vi "Host_spb.vi"   [LabVIEW 2018]
uses:
  <vilib>/userdefined/High Color/nirio_resource_hc.ctl
  <instrlib>/niDMM/nidmm.llb/niDMM Function.ctl
  <instrlib>/niDMM/nidmm.llb/niDMM Resolution in Digits.ctl
  <instrlib>/niDCPower/nidcpower.llb/niDCPower Measurement Type.ctl
  <instrlib>/niDMM/nidmm.llb/niDMM Configure Measurement Digits.vi
  <vilib>/FPGAPlugInAG/PXI-7953R/niLvFpga_Open_PXI-7953R.vi
  <vilib>/rvi/interface/common/dynamic/niFpgaDynamicAddResources.vi
  <vilib>/FPGAPlugInAG/Dynamic/niLvFpga_Reset_Dynamic.vi
  <vilib>/FPGAPlugInAG/Dynamic/niLvFpga_Run_Dynamic.vi
  <vilib>/Utility/error.llb/Error Cluster From Error Code.vi
  <vilib>/rvi/errors/niLvFpgaAdjustHostInterfaceError.vi
  <vilib>/FPGAPlugInAG/Dynamic/niLvFpga_Abort_Dynamic.vi
  <vilib>/rvi/interface/nirviOpenFPGA/nirviOpenFPGA.xnode
  <vilib>/rvi/interface/nirviMethod/nirviMethod.xnode
  <vilib>/rvi/interface/nirviReadWriteControl/nirviReadWriteControl.xnode
  NiFpgaLv.dll
  <vilib>/rvi/interface/Simulation/niFpgaSimulationCallBeginRW.vi
  <vilib>/FPGAPlugInAG/Dynamic/niLvFpga_ReadFifo_Dynamic.vi
  <vilib>/rvi/errors/niLvFpgaMergeErrorWithErrorCode.vi
types:
  T1 = enum16{"open", "replace", "create", "open or create", "replace or create", "replace or create with confirmation"}
  T2 = typedef "niDMM Function.ctl" = enum16{"DC Volts", "AC Volts", "DC Current", "AC Current", "2-wire Resistance", "4-wire Resistance", "Diode", "Frequency", "Period", "AC Volts DC Coupled", "Capacitance", "Inductance", "Temperature"}
  T3 = typedef "niDMM Resolution in Digits.ctl" = dbl
  T4 = cluster{"Global Rectangle":i32[], "Contours":cluster{"Contour Type":u32, "ROI Type":u32, "Points":i32[]}[]}
  T5 = cluster{"Contour Type":u32, "ROI Type":u32, "Points":i32[]}[]
  T6 = cluster{"Contour Type":u32, "ROI Type":u32, "Points":i32[]}
  T7 = typedef "IMAQ Image.ctl" = refnum<image>
  T8 = enum16{"Configuration", "MUX", "RED PGA", "GREEN PGA", "BLUE PGA", "RED OFF", "GREEN OFF", "BLUE OFF"}
  T9 = typedef "Image Type" = u32
  T10 = typedef "niDCPower Measurement Type.ctl" = i32
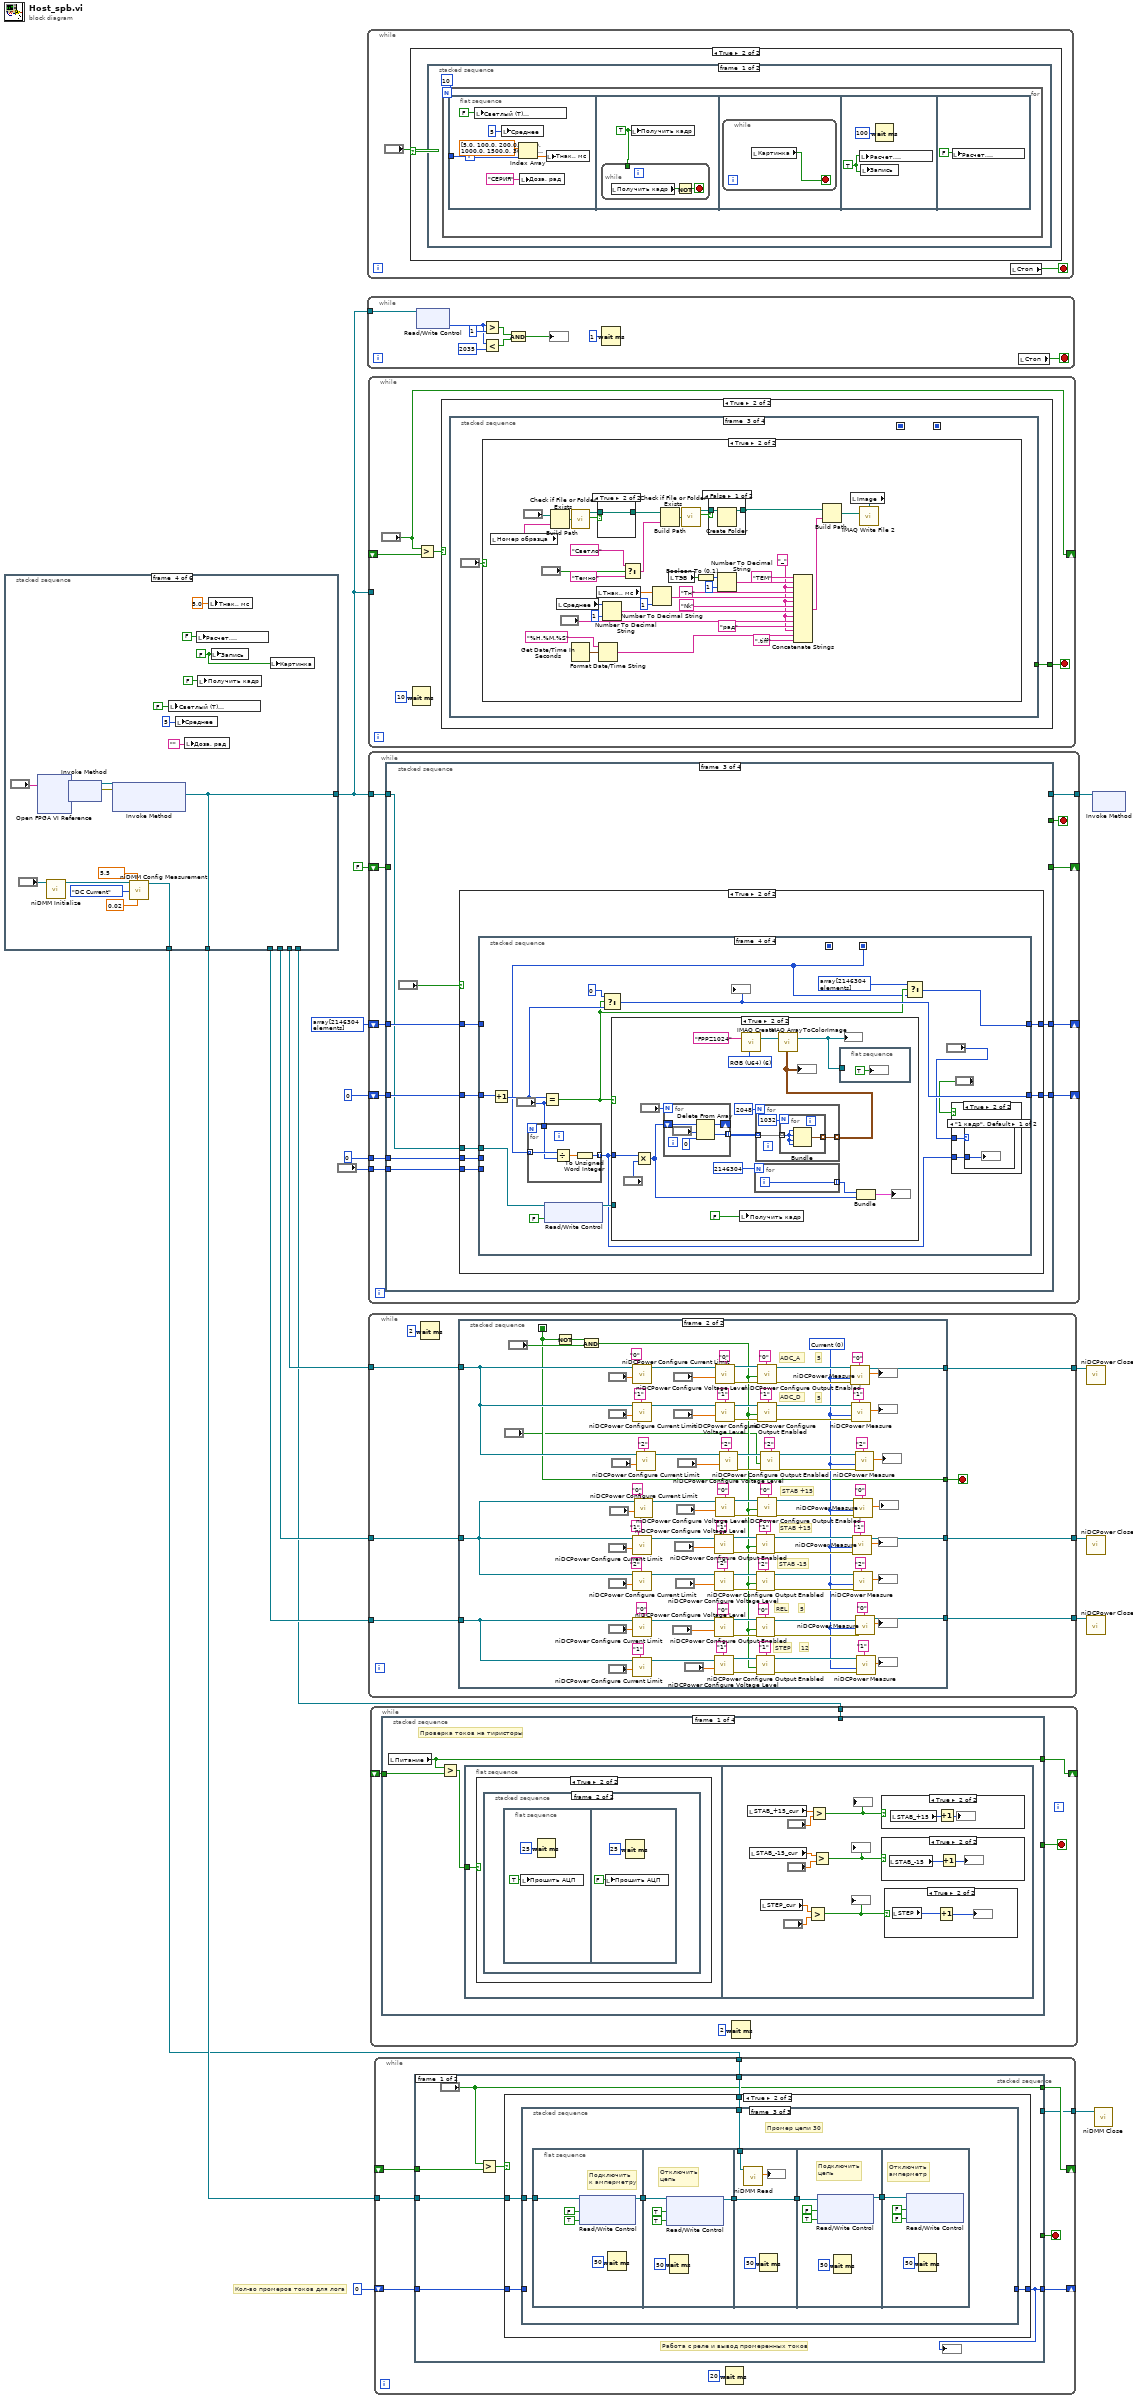
[diagram p0: block diagram]
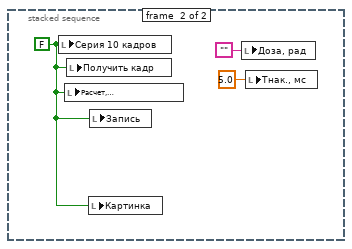
[diagram p3: hidden frame]
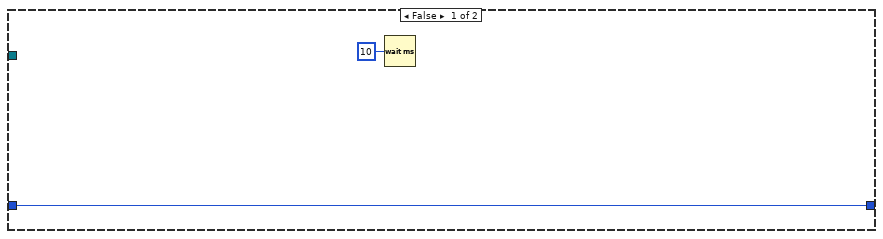
[diagram p4: hidden frame]
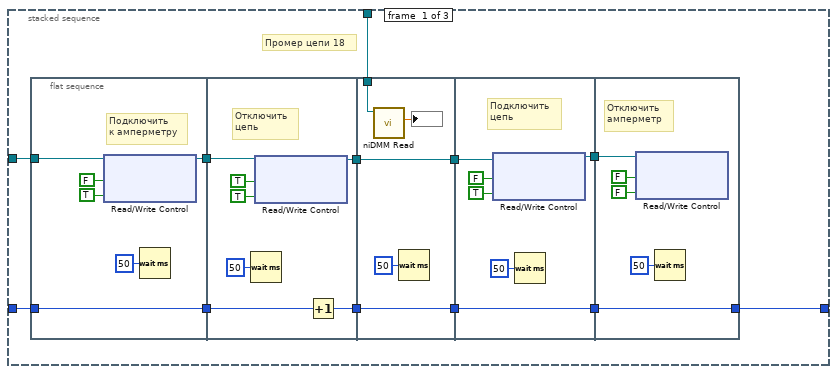
[diagram p5: hidden frame]
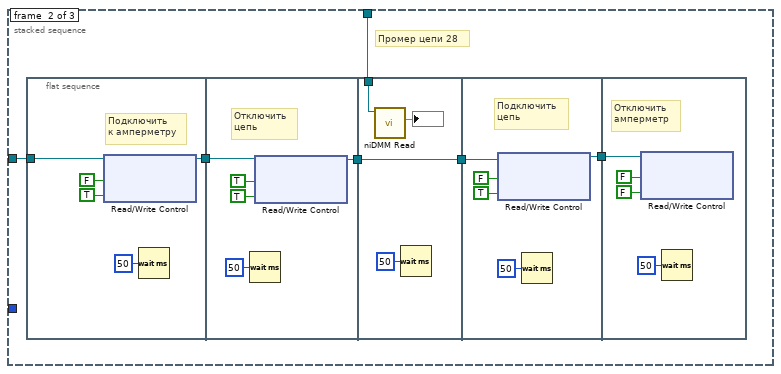
[diagram p6: hidden frame]
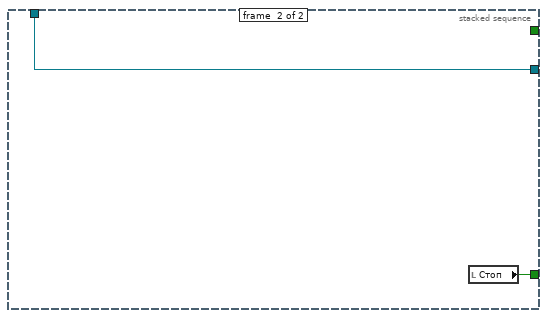
[diagram p7: hidden frame]
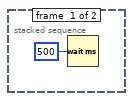
[diagram p9: hidden frame]
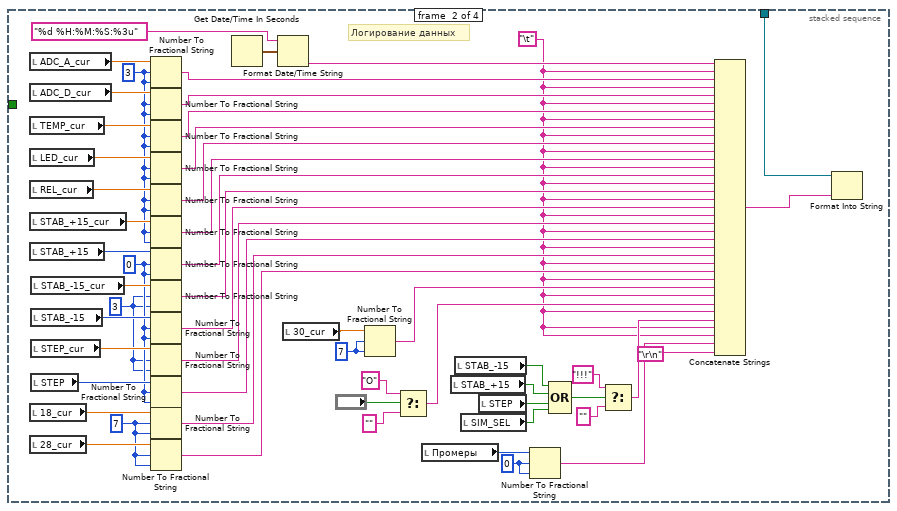
[diagram p13: hidden frame]
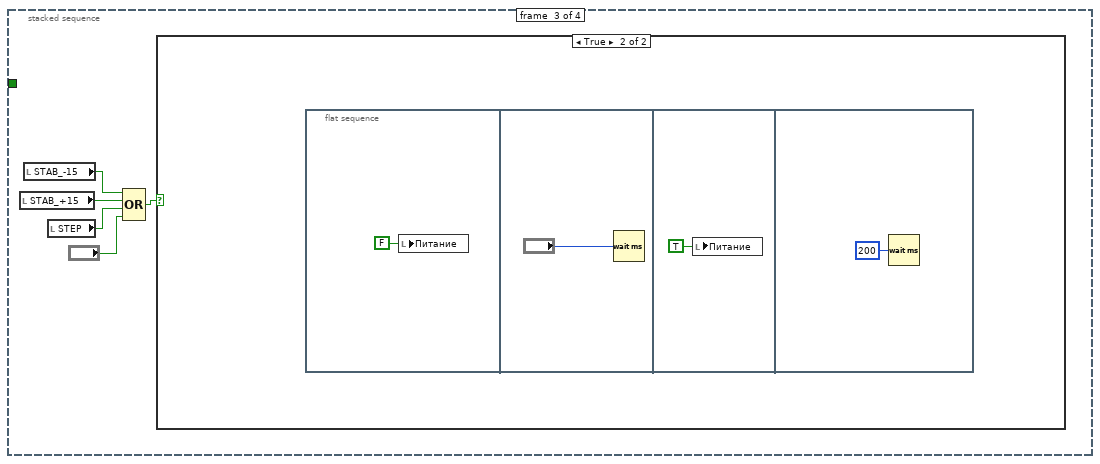
[diagram p14: hidden frame]
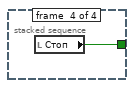
[diagram p16: hidden frame]
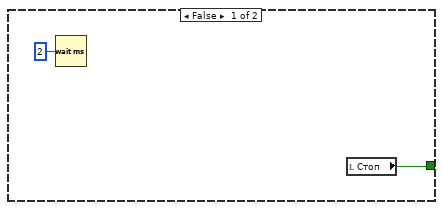
[diagram p17: hidden frame]
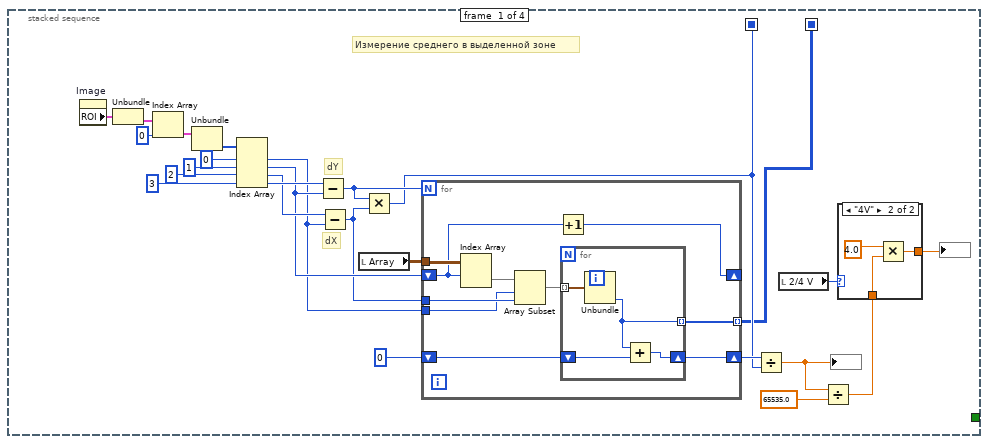
[diagram p18: hidden frame]
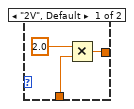
[diagram p19: hidden frame]
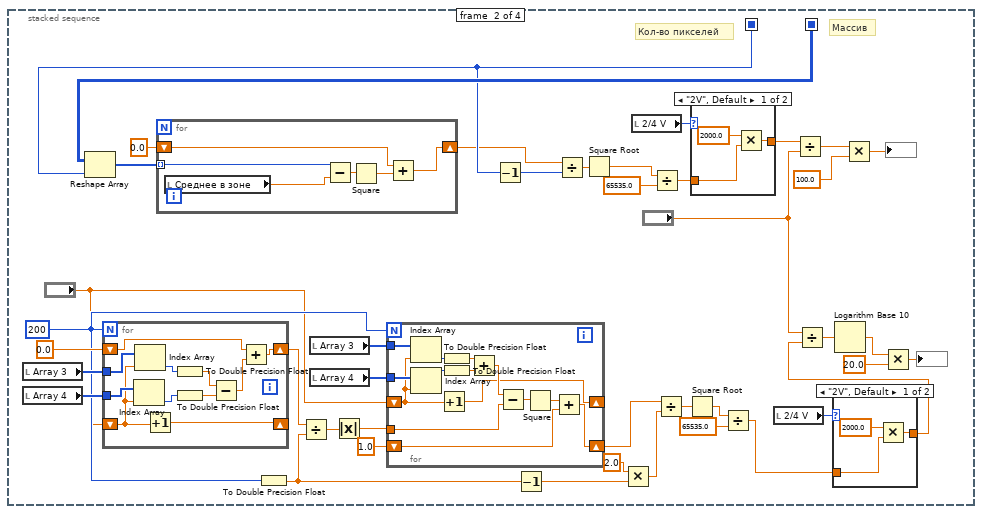
[diagram p20: hidden frame]
diagram:
  # "Кол-во промеров токов для лога"
  n1 = stacked-sequence {
    tunnel: [_ _ _ w73 _ _] -> w1
    tunnel: [_ _ _ _ w86 _] -> w18
    tunnel: [_ _ _ _ w85 _] -> w17
    tunnel: [_ _ _ _ w84 _] -> w16
    tunnel: [_ _ _ w75 _ _] -> w5
    tunnel: [_ _ _ w73 _ _] -> w6
    tunnel: [_ _ w23 _ _ _] -> w3
    frame #0 {
      n2 = call "Begin.vi"() -> ("Номер образца 2"=→"?":string)  [unwired: 11 in]
    }
    frame #1 {
      w21 = u8 0 ("Кол-во кадров")
      w20 = FALSE ("Стоп")
      # "Обнуление тиристоров"
      # "Отжатие всех кнопок управления"
      n3 = local write "Кол-во кадров"(w21) -> ()
      n4 = local write "STAB_+15"(w21) -> ()
      n5 = local write "STAB_-15"(w21) -> ()
      n6 = local write "STEP"(w21) -> ()
      n7 = local write "Стоп"(w20) -> ()
      n8 = local write "STAB_+15"(w20) -> ()
      n9 = local write "Питание"(w20) -> ()
      n10 = local write "STAB_-15"(w20) -> ()
      n11 = local write "STEP"(w20) -> ()
      n12 = local write "Линейки"(w20) -> ()
    }
    frame #2 {
      w26 = "\t"
      # "Инициализаци первой строки лога по токам"
      n13 = local read "Номер образца"() -> (w53:string)
      n14 = Build Path(base path="?", name or relative path=w53) -> (appended path=w55:path)
      n15 = Get Date/Time In Seconds() -> (seconds since 1Jan1904=w48:timestamp)
      n16 = call <vilib>:"Check if File or Folder Exists.vi"("path"=w55) -> ("file or folder exists?"=w56:bool, "dup path"=w57:path)  [unwired: 8 in, 1 out]
      n17 = Format Date/Time String(time format string (%c)="%d %H.%M.%S", seconds (now)=w48) -> (date/time string=w45:string)  [unwired: 1 in]
      n18 = case shown="False" w56 {
        tunnel: w57 -> [w63 w64]
        tunnel: [w62 w64] -> w22
        frame False {
          n19 = Create Folder(path (use dialog)=w63) -> (created path=w62:path)  [unwired: 2 in, 2 out]
        }
        frame True {
        }
      }
      n20 = Concatenate Strings(w45, ".xls" ("string")) -> (w43:string)
      n21 = Build Path(base path=w22, name or relative path=w43) -> (appended path=w46:path)
      n22 = Open/Create/Replace File(file path (use dialog)=w46, operation (0:open)=T1."open or create", access (0:read/write)=enum16{"read/write", "read-only", "write-only"}."read/write") -> (refnum out=w49:refnum<file>)  [unwired: 3 in, 2 out]
      n23 = case shown="True" TRUE {
        tunnel: w49 -> [w58 w61]
        tunnel: [w58 w59] -> w42
        frame False {
        }
        frame True {
          n24 = Set File Position(refnum=w61, from (0:start)=enum16{"start", "end", "current"}."end") -> (refnum out=w59:refnum<file>)  [unwired: 2 in, 1 out]
        }
      }
      n25 = Format Into String(initial string=w42, "Time" ("input 1"), w26, "ADC_A_cur" ("input 1"), w26, "ADC_D_cur" ("input 1"), w26, "TEM_cur" ("input 1"), w26, "LED_cur" ("input 1"), w26, "RELAY_cur" ("input 1"), w26, "ST+15_cur" ("input 1"), w26, "ST+15_q" ("input 1"), w26, "ST-15_cur" ("input 1"), w26, "ST-15_q" ("input 1"), w26, "STEP_cur" ("input 1"), w26, "STEP_q" ("input 1"), w26, "18_cur" ("input 1"), w26, "28_cur" ("input 1"), w26, "30_cur" ("input 1"), w26, "Облучение" ("input 1"), "\r\n") -> (resulting string=w23:refnum<file>)  [unwired: 2 in, 1 out]
    }
    frame #3 {
      w65 = FALSE ("Запись")
      w76 = T3 5.5 items=["3 1/2"=3.5, "4 1/2"=4.5, "5 1/2"=5.5, "6 1/2"=6.5, "7 1/2"=7.5] ("Resolution in Digits")
      n26 = xnode "Open FPGA VI Reference"("resource name"="?") -> ("FPGA VI Reference Out"=w83:refnum<k20>, "error out"=w81:errorcluster)  [unwired: 1 in]
      n27 = call <instrlib>:"niDMM Initialize.vi"("Instrument Descriptor"="?") -> ("instrument handle out"=w78:refnum<k15>)  [unwired: 9 in, 1 out]
      n28 = xnode "Invoke Method"("FPGA VI Reference In"=w83, "error in"=w81) -> ("FPGA VI Reference Out"=w80:refnum<k20>, "error out"=w82:errorcluster)
      n29 = xnode "Invoke Method"("FPGA VI Reference In"=w80, "error in"=w82) -> ("FPGA VI Reference Out"=w73:refnum<k20>)  [unwired: 1 in, 1 out]
      n30 = call-poly <instrlib>:"niDMM Config Measurement.vi"("Range"=0.02, "Resolution in Digits"=w76, "Function"=niDMM_Function."DC Current", "instrument handle"=w78) -> ("instrument handle out"=w75:refnum<k15>)  [unwired: 6 in, 1 out]
      n31 = local write "Светлый (T)\nТемный (F)"(FALSE ("Светлый (T)\nТемный (F)")) -> ()
      n32 = local write "Среднее"(u8 5 ("Среднее")) -> ()
      n33 = local write "Доза, рад"("") -> ()
      n34 = local write "Расчет,\nзапись (?)"(FALSE ("Расчет,\nзапись (?)")) -> ()
      n35 = local write "Получить кадр"(FALSE ("Получить кадр")) -> ()
      n36 = local write "Tнак., мс"(5.0 ("Tнак., мс")) -> ()
      n37 = local write "Запись"(w65) -> ()
      n38 = local write "Картинка"(w65) -> ()
    }
    frame #4 {
      n39 = call <instrlib>:"niDCPower Initialize.vi"("resource name"="?") -> ("error out"=w96:errorcluster, "instrument handle out"=w99:refnum<k15>)  [unwired: 3 in, 6 out]
      n40 = call <instrlib>:"niDCPower Initialize.vi"("resource name"="?") -> ("error out"=w97:errorcluster, "instrument handle out"=w100:refnum<k15>)  [unwired: 3 in, 6 out]
      n41 = call <instrlib>:"niDCPower Initialize.vi"("resource name"="?") -> ("error out"=w98:errorcluster, "instrument handle out"=w101:refnum<k15>)  [unwired: 3 in, 6 out]
      n42 = call <instrlib>:"niDCPower Configure Voltage Level.vi"("error in (no error)"=w96, "voltage level"=0.0, "channel name"="0,1,2", "instrument handle"=w99) -> ("instrument handle out"=w84:refnum<k15>)  [unwired: 6 in, 1 out]
      n43 = call <instrlib>:"niDCPower Configure Voltage Level.vi"("error in (no error)"=w97, "voltage level"=0.0, "channel name"="0,1,2", "instrument handle"=w100) -> ("instrument handle out"=w85:refnum<k15>)  [unwired: 6 in, 1 out]
      n44 = call <instrlib>:"niDCPower Configure Voltage Level.vi"("error in (no error)"=w98, "voltage level"=0.0, "channel name"="0,1", "instrument handle"=w101) -> ("instrument handle out"=w86:refnum<k15>)  [unwired: 6 in, 1 out]
    }
    frame #5 {
      # "Здесь надо расписать данные, которые идут в лог!"
    }
  }
  n45 = while {
    stop <- w102 stop-if-true
    n46 = case shown="True" "?" {
      frame False {
      }
      frame True {
        n47 = stacked-sequence {
          frame #0 {
            n48 = for {
              N: 10 -> [_]
              i -> [w105]
              n49 = flat-sequence {
                tunnel: w105 -> [w110]
                frame #0 {
                  n50 = local write "Светлый (T)\nТемный (F)"(FALSE ("Светлый (T)\nТемный (F)")) -> ()
                  n51 = local write "Среднее"(u8 5 ("Среднее")) -> ()
                  n52 = Index Array(array=dbl[] [5.0, 100.0, 200.0, 500.0, 1000.0, 1500.0, 3000.0, 3500.0, 4500.0, 5000.0], index=w110) -> (element=w107:dbl)
                  n53 = local write "Доза, рад"("СЕРИЯ" ("Доза, рад")) -> ()
                  n54 = local write "Tнак., мс"(w107) -> ()
                }
                frame #1 {
                  w112 = TRUE ("Получить кадр")
                  n55 = while {
                    tunnel: w112 -> [_]
                    stop <- w114 stop-if-true
                    n56 = local read "Получить кадр"() -> (w113:bool)
                    n57 = Not(x=w113) -> (.not. x?=w114:bool)
                  }
                  n58 = local write "Получить кадр"(w112) -> ()
                }
                frame #2 {
                  n59 = while {
                    stop <- w115 stop-if-true
                    n60 = local read "Картинка"() -> (w115:bool)
                  }
                }
                frame #3 {
                  w117 = TRUE ("Запись")
                  n61 = local write "Расчет,\nзапись (?)"(w117) -> ()
                  n62 = local write "Запись"(w117) -> ()
                  n63 = Wait (ms)(milliseconds to wait=u32 100) -> ()  [unwired: 1 out]
                }
                frame #4 {
                  n64 = local write "Расчет,\nзапись (?)"(FALSE) -> ()
                }
              }
            }
          }
          frame #1 {
            w119 = FALSE ("Серия 10 кадров")
            n65 = local write "Серия 10 кадров"(w119) -> ()
            n66 = local write "Расчет,\nзапись (?)"(w119) -> ()
            n67 = local write "Получить кадр"(w119) -> ()
            n68 = local write "Картинка"(w119) -> ()
            n69 = local write "Запись"(w119) -> ()
            n70 = local write "Доза, рад"("") -> ()
            n71 = local write "Tнак., мс"(5.0 ("Tнак., мс")) -> ()
          }
        }
      }
    }
    n72 = local read "Стоп"() -> (w102:bool)
  }
  n73 = while {
    tunnel: w1 -> [w129]
    stop <- w130 stop-if-true
    n74 = xnode "Read/Write Control"("FPGA VI Reference In"=w129) -> ("I"=w125:i32)  [unwired: 1 in, 2 out]
    n75 = Greater?(x=w125, y=1) -> (0:w128:bool)
    n76 = Less?(x=w125, y=2035) -> (x < y?=w127:bool)
    n77 = And(x=w128, y=w127) -> (x .and. y?=→"?":bool)
    n78 = Wait (ms)(milliseconds to wait=u32 1) -> ()  [unwired: 1 out]
    n79 = local read "Стоп"() -> (w130:bool)
  }
  n80 = while {
    shift-right: ["?"] -> _
    shift-left: _ -> [w135]
    tunnel: w1 -> [_]
    stop <- w131 stop-if-true
    n81 = Wait (ms)(milliseconds to wait=u32 10) -> ()  [unwired: 1 out]
    n82 = Greater?(x="?", y=w135) -> (0:w134:bool)
    n83 = case shown="True" w134 {
      tunnel: [w136 w138] -> w131
      frame False {
        n84 = Wait (ms)(milliseconds to wait=u32 2) -> ()  [unwired: 1 out]
        n85 = local read "Стоп"() -> (w136:bool)
      }
      frame True {
        n86 = stacked-sequence {
          seq-local: [w140 _ _ _] -> [_ w221 _ _]
          seq-local: [w139 _ _ _] -> [_ w223 _ _]
          tunnel: [_ _ _ w314] -> w138
          frame #0 {
            # "Измерение среднего в выделенной зоне"
            # "dX"
            # "dY"
            n87 = property on="Image" class="ImageControl"() -> ("ROI"=w163:T4)  [unwired: 2 in, 2 out]
            n88 = Unbundle(w163) -> ("Contours"=w162:T5)  [unwired: 1 out]
            n89 = Index Array(array=w162, index=0) -> (element=w160:T6)
            n90 = Unbundle(w160) -> ("Points"=w159:i32[])  [unwired: 2 out]
            n91 = Index Array(array=w159, index #1=0 ("index"), index #2=1 ("index"), index #3=2 ("index"), index #4=3 ("index")) -> (element #1=w148:i32, element #2=w151:i32, element #3=w153:i32, element #4=w154:i32)
            n92 = Subtract(x=w154, y=w151) -> (x-y=w152:i32)
            n93 = Subtract(x=w153, y=w148) -> (x-y=w149:i32)
            n94 = local read "Array"() -> (w150:cluster{u64, u64, u64, u64}[][])
            n95 = Multiply(x=w152, y=w149) -> (x*y=w140:i32)
            n96 = for {
              N: w152 -> [_]
              shift-right: [w171] -> _
              shift-left: w151 -> [w172]
              tunnel: w150 -> [w179]
              tunnel: w149 -> [w177]
              tunnel: w148 -> [w176]
              shift-right: [w173] -> w146
              shift-left: 0 -> [w174]
              tunnel: [w170] -> w139 mode=indexing
              n97 = Index Array(array=w179, index (row)=w172) -> (element=w178:cluster{u64, u64, u64, u64}[])  [unwired: 1 in]
              n98 = Array Subset(array=w178, index=w176, length=w177) -> (w175:cluster{u64, u64, u64, u64}[])
              n99 = Increment(x=w172) -> (x+1=w171:i32)
              n100 = for {
                tunnel: w175 -> [w183] mode=indexing
                shift-right: [w182] -> w173
                shift-left: w174 -> [w181]
                tunnel: [w180] -> w170 mode=indexing
                n101 = Unbundle(w183) -> (w180:u64)  [unwired: 3 out]
                n102 = Add(x=w180, y=w181) -> (x+y=w182:u64)
              }
            }
            n103 = Divide(x=w146, y=w140) -> (x/y=w144:dbl)
            "?" <- w144
            n104 = local read "2/4 V"() -> (w145:enum16{"2V", "4V"})
            n105 = Divide(x=w144, y=65535.0) -> (x/y=w142:dbl)
            n106 = case shown="\"4V\"" w145 {
              tunnel: w142 -> [w166 w168]
              tunnel: [w164 w167] -> w141
              frame "2V", Default {
                n107 = Multiply(x=2.0, y=w166) -> (x*y=w164:dbl)
              }
              frame "4V" {
                n108 = Multiply(x=4.0, y=w168) -> (x*y=w167:dbl)
              }
            }
            "?" <- w141
          }
          frame #1 {
            w187 = 200
            # "Массив"
            # "Кол-во пикселей"
            n109 = local read "Array 3"() -> (w188:u16[])
            n110 = local read "Array 4"() -> (w189:u16[])
            n111 = Reshape Array(w223, w221) -> (w222:u64[])
            n112 = for {
              N: w187 -> [_]
              shift-right: [w254] -> w193
              shift-left: 0.0 -> [w252]
              shift-right: [w246] -> _
              shift-left: "?" -> [w249]
              tunnel: w189 -> [w250]
              tunnel: w188 -> [w251]
              n113 = Index Array(array=w250, index=w249) -> (element=w247:u16)
              n114 = Index Array(array=w251, index=w249) -> (element=w248:u16)
              n115 = Increment(x=w249) -> (x+1=w246:dbl)
              n116 = To Double Precision Float(number=w248) -> (double precision float=w256:dbl)
              n117 = To Double Precision Float(number=w247) -> (double precision float=w255:dbl)
              n118 = Subtract(x=w256, y=w255) -> (x-y=w253:dbl)
              n119 = Add(x=w252, y=w253) -> (x+y=w254:dbl)
            }
            n120 = for {
              tunnel: w222 -> [w264] mode=indexing
              shift-right: [w265] -> w220
              shift-left: 0.0 -> [w266]
              n121 = local read "Среднее в зоне"() -> (w263:dbl)
              n122 = Subtract(x=w264, y=w263) -> (x-y=w268:dbl)
              n123 = Square(x=w268) -> (x^2=w267:dbl)
              n124 = Add(x=w266, y=w267) -> (x+y=w265:dbl)
            }
            n125 = To Double Precision Float(number=w187) -> (double precision float=w192:dbl)
            n126 = Divide(x=w193, y=w192) -> (x/y=w191:dbl)
            n127 = local read "Array 3"() -> (w186:u16[])
            n128 = local read "Array 4"() -> (w185:u16[])
            n129 = Absolute Value(x=w191) -> (abs(x)=w190:dbl)
            n130 = for {
              N: w187 -> [_]
              shift-right: [w241] -> w206
              shift-left: 1.0 -> [w242]
              tunnel: w190 -> [w244]
              shift-right: [w235] -> _
              shift-left: "?" -> [w232]
              tunnel: w186 -> [w237]
              tunnel: w185 -> [w233]
              n131 = Index Array(array=w237, index=w232) -> (element=w238:u16)
              n132 = Index Array(array=w233, index=w232) -> (element=w234:u16)
              n133 = Increment(x=w232) -> (x+1=w235:dbl)
              n134 = To Double Precision Float(number=w238) -> (double precision float=w240:dbl)
              n135 = To Double Precision Float(number=w234) -> (double precision float=w239:dbl)
              n136 = Add(x=w240, y=w239) -> (x+y=w245:dbl)
              n137 = Subtract(x=w245, y=w244) -> (x-y=w236:dbl)
              n138 = Square(x=w236) -> (x^2=w243:dbl)
              n139 = Add(x=w243, y=w242) -> (x+y=w241:dbl)
            }
            n140 = Decrement(x=w221) -> (x-1=w224:i32)
            n141 = Decrement(x=w192) -> (x-1=w204:dbl)
            n142 = Divide(x=w220, y=w224) -> (x/y=w225:dbl)
            n143 = Square Root(x=w225) -> (sqrt(x)=w215:dbl)
            n144 = Multiply(x=2.0 ("y"), y=w204) -> (x*y=w203:dbl)
            n145 = local read "2/4 V"() -> (w217:enum16{"2V", "4V"})
            n146 = Divide(x=w215, y=65535.0) -> (x/y=w214:dbl)
            n147 = Divide(x=w206, y=w203) -> (x/y=w202:dbl)
            n148 = Square Root(x=w202) -> (sqrt(x)=w199:dbl)
            n149 = case shown="\"2V\", Default" w217 {
              tunnel: [w258 w261] -> w213
              tunnel: w214 -> [w257 w260]
              frame "2V", Default {
                n150 = Multiply(x=2000.0, y=w257) -> (x*y=w258:dbl)
              }
              frame "4V" {
                n151 = Multiply(x=4000.0, y=w260) -> (x*y=w261:dbl)
              }
            }
            n152 = Divide(x=w199, y=65535.0) -> (x/y=w197:dbl)
            n153 = local read "2/4 V"() -> (w196:enum16{"2V", "4V"})
            n154 = Divide(x=w213, y="?") -> (x/y=w212:dbl)
            n155 = case shown="\"2V\", Default" w196 {
              tunnel: [w227 w230] -> w195
              tunnel: w197 -> [w226 w229]
              frame "2V", Default {
                n156 = Multiply(x=2000.0, y=w226) -> (x*y=w227:dbl)
              }
              frame "4V" {
                n157 = Multiply(x=4000.0, y=w229) -> (x*y=w230:dbl)
              }
            }
            n158 = Divide(x="?", y=w195) -> (x/y=w200:dbl)
            n159 = Logarithm Base 10(1:w200) -> (0:w210:dbl)
            n160 = Multiply(x=w212, y=100.0) -> (x*y=→"?":dbl)
            n161 = Multiply(x=w210, y=20.0) -> (x*y=→"?":dbl)
          }
          frame #2 {
            n162 = case shown="True" "?" {
              frame False {
                n163 = Wait (ms)(milliseconds to wait=u32 5) -> ()  [unwired: 1 out]
              }
              frame True {
                w277 = "_" ("element")
                n164 = local read "Номер образца"() -> (w272:string)
                n165 = Build Path(base path="?", name or relative path=w272) -> (appended path=w300:path)
                n166 = local read "Среднее"() -> (w282:u8)
                n167 = call <vilib>:"Check if File or Folder Exists.vi"("path"=w300) -> ("file or folder exists?"=w301:bool, "dup path"=w302:path)  [unwired: 8 in, 1 out]
                n168 = Get Date/Time In Seconds() -> (seconds since 1Jan1904=w275:timestamp)
                n169 = local read "Tнак., мс"() -> (w285:dbl)
                n170 = case shown="True" w301 {
                  tunnel: w302 -> [w312 w313]
                  tunnel: [w311 w313] -> w296
                  frame False {
                    n171 = Create Folder(path (use dialog)=w312) -> (created path=w311:path)  [unwired: 2 in, 2 out]
                  }
                  frame True {
                  }
                }
                n172 = Format Date/Time String(time format string (%c)="%H.%M.%S", seconds (now)=w275) -> (date/time string=w274:string)  [unwired: 1 in]
                n173 = Number To Decimal String(number=w282, width (-)=i16 1) -> (decimal integer string=w280:string)
                n174 = Select(t="Светло", s="?", f="Темно") -> (s? t:f=w295:string)
                n175 = Number To Decimal String(number=w285, width (-)=i16 1) -> (decimal integer string=w284:string)
                n176 = Build Path(base path=w296, name or relative path=w295) -> (appended path=w299:path)
                n177 = local read "ТЭБ"() -> (w292:bool)
                n178 = call <vilib>:"Check if File or Folder Exists.vi"("path"=w299) -> ("file or folder exists?"=w298:bool, "dup path"=w297:path)  [unwired: 8 in, 1 out]
                n179 = Boolean To (0,1)(Boolean=w292) -> (0, 1=w290:i16)
                n180 = case shown="False" w298 {
                  tunnel: w297 -> [w309 w310]
                  tunnel: [w308 w310] -> w271
                  frame False {
                    n181 = Create Folder(path (use dialog)=w309) -> (created path=w308:path)  [unwired: 2 in, 2 out]
                  }
                  frame True {
                  }
                }
                n182 = Number To Decimal String(number=w290, width (-)=i16 1) -> (decimal integer string=w288:string)
                n183 = Concatenate Strings("ТЕМ" ("element"), w288, w277, "Тн" ("element"), w284, w277, "Nk" ("element"), w280, w277, "?", "рад" ("element"), w277, w274, ".tiff" ("element")) -> (w294:string)
                n184 = Build Path(base path=w271, name or relative path=w294) -> (appended path=w293:path)
                n185 = local read "Image"() -> (w307:T7)
                n186 = call-poly "IMAQ Write File 2"("File Path"=w293, "Image"=w307) -> ()  [unwired: 8 in, 2 out]
              }
            }
          }
          frame #3 {
            n187 = local read "Стоп"() -> (w314:bool)
          }
        }
      }
    }
  }
  n188 = while {
    tunnel: w1 -> [w325]
    tunnel: [w323] -> w12
    tunnel: u32 0 -> [w322]
    tunnel: "?" -> [w321]
    shift-right: [w319] -> _
    shift-left: FALSE -> [w320]
    shift-right: [w317] -> _
    shift-left: u8 0 -> [w318]
    shift-right: [w316] -> _
    shift-left: u64[] array[2146304 elements] -> [w315]
    stop <- w324 stop-if-true
    n189 = stacked-sequence {
      tunnel: w325 -> [w353 w370 w556 w726]
      tunnel: [_ _ _ "?"] -> w324
      tunnel: [_ _ _ w725] -> w323
      tunnel: w322 -> [_ _ w563 _]
      tunnel: w321 -> [_ _ w562 _]
      tunnel: w320 -> [_ w372 _ _]
      tunnel: [_ "?" _ _] -> w319
      tunnel: w318 -> [_ _ w561 _]
      tunnel: [_ _ w560 _] -> w317
      tunnel: [_ _ w559 _] -> w316
      tunnel: w315 -> [_ _ w558 _]
      frame #0 {
        n190 = local read "Питание"() -> (w350:bool)
        n191 = And(x="?", y=w350) -> (x .and. y?=w352:bool)
        n192 = xnode "Read/Write Control"("FPGA VI Reference In"=w353, "2"="?", "4"="?", "1800"="?", "10"="?", "30"="?", "Строка триггер"="?", "Горизонталы"="?", "H1_1"="?", "H1_2"="?", "H2_1"="?", "H2_2"="?", "H3_1"="?", "H3_2"="?", "RG_1"="?", "RG_2"="?", "48"="?", "После H, мкс"="?", "CDS1_1"="?", "CDS1_2"="?", "CDS2_1"="?", "CDS2_2"="?", "ADC_1"="?", "ADC_2"="?", "Задержка после переноса строки, мкс"="?", "S3_1"="?", "S3_2"="?", "S2_1"="?", "S2_2"="?", "S1_1"="?", "S1_2"="?", "Сколько строк?"="?", "Линейки"=w352) -> ()  [unwired: 1 in, 2 out]
        n193 = Multiply(x="?", y=40000.0) -> (x*y=w328:dbl)
        n194 = Multiply(x="?", y=40000.0) -> (x*y=w326:dbl)
        n195 = xnode "Read/Write Control"("FPGA VI Reference In"=w353, "Свет от"=u32 0, "Свет до"=w326, "Задержка"=w328, "Свет"="?") -> ()  [unwired: 1 in, 2 out]
      }
      frame #1 {
        n196 = Greater?(x="?", y=w372) -> (0:w369:bool)
        n197 = case shown="True" w369 {
          tunnel: w370 -> [_ w373]
          frame False {
          }
          frame True {
            n198 = stacked-sequence {
              tunnel: w373 -> [w398 w447 w496 w527]
              frame #0 {
                w394 = TRUE ("element")
                w395 = FALSE
                # "8"
                # "0"
                # "Configuration"
                n199 = case shown="\"3CH\", Default" "?" {
                  tunnel: [TRUE FALSE] -> w393
                  frame "3CH", Default {
                  }
                  frame "1CH" {
                  }
                }
                n200 = case shown="\"4V\"" "?" {
                  tunnel: [FALSE TRUE] -> w391
                  frame "2V", Default {
                  }
                  frame "4V" {
                  }
                }
                n201 = xnode "Read/Write Control"("FPGA VI Reference In"=w375, "Read(T)/Write(F)"=TRUE) -> ("FPGA VI Reference Out"=w381:refnum<k20>, "error out"=w380:errorcluster)  [unwired: 1 in]
                n202 = xnode "Read/Write Control"("FPGA VI Reference In"=w398, "Enum"=T8."Configuration") -> ("FPGA VI Reference Out"=w385:refnum<k20>)  [unwired: 1 in, 1 out]
                n203 = xnode "Read/Write Control"("FPGA VI Reference In"=w385, "Read(T)/Write(F)"=FALSE) -> ("FPGA VI Reference Out"=w383:refnum<k20>)  [unwired: 1 in, 1 out]
                n204 = Build Array(w395, w395, w395, w394, w394, w393, w394, w391, FALSE) -> (w396:bool[])
                n205 = flat-sequence {
                  tunnel: w381 -> [w410]
                  tunnel: w380 -> [w409]
                  tunnel: [w408] -> w379
                  tunnel: [w407] -> w378
                  frame #0 {
                    n206 = xnode "Read/Write Control"("FPGA VI Reference In"=w410, "error in"=w409, "Конфигурация"=TRUE) -> ("FPGA VI Reference Out"=w408:refnum<k20>, "error out"=w407:errorcluster)
                    n207 = Wait (ms)(milliseconds to wait=u32 10) -> ()  [unwired: 1 out]
                  }
                }
                n208 = Reverse 1D Array(array=w396) -> (reversed array=w388:bool[])
                n209 = xnode "Read/Write Control"("FPGA VI Reference In"=w383, "Write Data"=w388) -> ("FPGA VI Reference Out"=w387:refnum<k20>)  [unwired: 1 in, 1 out]
                n210 = flat-sequence {
                  tunnel: w379 -> [w404]
                  tunnel: w378 -> [w403]
                  tunnel: [w401] -> w377
                  tunnel: [w400] -> w376
                  frame #0 {
                    n211 = xnode "Read/Write Control"("FPGA VI Reference In"=w404, "error in"=w403, "Конфигурация"=FALSE) -> ("FPGA VI Reference Out"=w401:refnum<k20>, "error out"=w400:errorcluster)
                    n212 = Wait (ms)(milliseconds to wait=u32 10) -> ()  [unwired: 1 out]
                  }
                }
                n213 = flat-sequence {
                  tunnel: w387 -> [w418]
                  tunnel: [w416] -> w386
                  frame #0 {
                    n214 = xnode "Read/Write Control"("FPGA VI Reference In"=w418, "Конфигурация"=TRUE) -> ("FPGA VI Reference Out"=w416:refnum<k20>)  [unwired: 1 in, 1 out]
                    n215 = Wait (ms)(milliseconds to wait=u32 10) -> ()  [unwired: 1 out]
                  }
                }
                n216 = xnode "Read/Write Control"("FPGA VI Reference In"=w377, "error in"=w376) -> ("READ"=→"?":bool[])  [unwired: 2 out]
                n217 = flat-sequence {
                  tunnel: w386 -> [w414]
                  tunnel: [w412] -> w375
                  frame #0 {
                    n218 = xnode "Read/Write Control"("FPGA VI Reference In"=w414, "Конфигурация"=FALSE) -> ("FPGA VI Reference Out"=w412:refnum<k20>)  [unwired: 1 in, 1 out]
                    n219 = Wait (ms)(milliseconds to wait=u32 10) -> ()  [unwired: 1 out]
                  }
                }
              }
              frame #1 {
                # "GREEN OFF"
                n220 = xnode "Read/Write Control"("FPGA VI Reference In"=w434, "Read(T)/Write(F)"=TRUE) -> ("FPGA VI Reference Out"=w445:refnum<k20>, "error out"=w444:errorcluster)  [unwired: 1 in]
                n221 = case shown="\"-\", Default" "?" {
                  tunnel: [TRUE FALSE] -> w425
                  frame "-", Default {
                  }
                  frame "+" {
                  }
                }
                n222 = Quotient & Remainder(x="?", y=1.171875) -> (floor(x/y)=w430:dbl)  [unwired: 1 out]
                n223 = xnode "Read/Write Control"("FPGA VI Reference In"=w447, "Enum"=T8."GREEN OFF") -> ("FPGA VI Reference Out"=w438:refnum<k20>, "error out"=w437:errorcluster)  [unwired: 1 in]
                n224 = Subtract(x=w430, y=1.0) -> (x-y=w427:dbl)
                n225 = flat-sequence {
                  tunnel: w445 -> [w468]
                  tunnel: w444 -> [w467]
                  tunnel: [w466] -> w443
                  tunnel: [w465] -> w442
                  frame #0 {
                    n226 = xnode "Read/Write Control"("FPGA VI Reference In"=w468, "error in"=w467, "Конфигурация"=TRUE) -> ("FPGA VI Reference Out"=w466:refnum<k20>, "error out"=w465:errorcluster)
                    n227 = Wait (ms)(milliseconds to wait=u32 10) -> ()  [unwired: 1 out]
                  }
                }
                n228 = To Unsigned Byte Integer(number=w427) -> (unsigned 8bit integer=w426:u8)
                n229 = xnode "Read/Write Control"("FPGA VI Reference In"=w438, "error in"=w437, "Read(T)/Write(F)"=FALSE) -> ("FPGA VI Reference Out"=w436:refnum<k20>)  [unwired: 1 out]
                n230 = Number To Boolean Array(number=w426) -> (Boolean array=w424:bool[])
                n231 = Reverse 1D Array(array=w424) -> (reversed array=w423:bool[])
                n232 = Build Array (concatenate)(w425, w423) -> (w428:bool[])
                n233 = xnode "Read/Write Control"("FPGA VI Reference In"=w436, "Write Data"=w428) -> ("FPGA VI Reference Out"=w449:refnum<k20>)  [unwired: 1 in, 1 out]
                n234 = flat-sequence {
                  tunnel: w443 -> [w458]
                  tunnel: w442 -> [w457]
                  tunnel: [w455] -> w441
                  tunnel: [w454] -> w440
                  frame #0 {
                    n235 = xnode "Read/Write Control"("FPGA VI Reference In"=w458, "error in"=w457, "Конфигурация"=FALSE) -> ("FPGA VI Reference Out"=w455:refnum<k20>, "error out"=w454:errorcluster)
                    n236 = Wait (ms)(milliseconds to wait=u32 10) -> ()  [unwired: 1 out]
                  }
                }
                n237 = flat-sequence {
                  tunnel: w449 -> [w472]
                  tunnel: [w470] -> w448
                  frame #0 {
                    n238 = xnode "Read/Write Control"("FPGA VI Reference In"=w472, "Конфигурация"=TRUE) -> ("FPGA VI Reference Out"=w470:refnum<k20>)  [unwired: 1 in, 1 out]
                    n239 = Wait (ms)(milliseconds to wait=u32 10) -> ()  [unwired: 1 out]
                  }
                }
                n240 = xnode "Read/Write Control"("FPGA VI Reference In"=w441, "error in"=w440) -> ("READ"=→"?":bool[])  [unwired: 2 out]
                n241 = flat-sequence {
                  tunnel: w448 -> [w462]
                  tunnel: [w460] -> w434
                  frame #0 {
                    n242 = xnode "Read/Write Control"("FPGA VI Reference In"=w462, "Конфигурация"=FALSE) -> ("FPGA VI Reference Out"=w460:refnum<k20>)  [unwired: 1 in, 1 out]
                    n243 = Wait (ms)(milliseconds to wait=u32 10) -> ()  [unwired: 1 out]
                  }
                }
              }
              frame #2 {
                w482 = FALSE
                # "GREEN PGA"
                n244 = xnode "Read/Write Control"("FPGA VI Reference In"=w494, "Read(T)/Write(F)"=TRUE) -> ("FPGA VI Reference Out"=w489:refnum<k20>, "error out"=w488:errorcluster)  [unwired: 1 in]
                n245 = Decrement(x="?") -> (x-1=w474:u8)
                n246 = Multiply(x=w474, y=378) -> (x*y=w476:i32)
                n247 = Multiply(x="?", y=5) -> (x*y=w479:i32)
                n248 = xnode "Read/Write Control"("FPGA VI Reference In"=w496, "Enum"=T8."GREEN PGA") -> ("FPGA VI Reference Out"=w493:refnum<k20>)  [unwired: 1 in, 1 out]
                n249 = Divide(x=w476, y=w479) -> (x/y=w480:dbl)
                n250 = Number To Boolean Array(number=w480) -> (Boolean array=w473:bool[])
                n251 = xnode "Read/Write Control"("FPGA VI Reference In"=w493, "Read(T)/Write(F)"=FALSE) -> ("FPGA VI Reference Out"=w492:refnum<k20>)  [unwired: 1 in, 1 out]
                n252 = flat-sequence {
                  tunnel: w489 -> [w510]
                  tunnel: w488 -> [w509]
                  tunnel: [w508] -> w487
                  tunnel: [w507] -> w486
                  frame #0 {
                    n253 = xnode "Read/Write Control"("FPGA VI Reference In"=w510, "error in"=w509, "Конфигурация"=TRUE) -> ("FPGA VI Reference Out"=w508:refnum<k20>, "error out"=w507:errorcluster)
                    n254 = Wait (ms)(milliseconds to wait=u32 10) -> ()  [unwired: 1 out]
                  }
                }
                n255 = Build Array (concatenate)(w482, w482, w482, w473) -> (w481:bool[])
                n256 = xnode "Read/Write Control"("FPGA VI Reference In"=w492, "Write Data"=w481) -> ("FPGA VI Reference Out"=w495:refnum<k20>)  [unwired: 1 in, 1 out]
                n257 = flat-sequence {
                  tunnel: w487 -> [w504]
                  tunnel: w486 -> [w503]
                  tunnel: [w501] -> w485
                  tunnel: [w500] -> w484
                  frame #0 {
                    n258 = xnode "Read/Write Control"("FPGA VI Reference In"=w504, "error in"=w503, "Конфигурация"=FALSE) -> ("FPGA VI Reference Out"=w501:refnum<k20>, "error out"=w500:errorcluster)
                    n259 = Wait (ms)(milliseconds to wait=u32 10) -> ()  [unwired: 1 out]
                  }
                }
                n260 = flat-sequence {
                  tunnel: [w517] -> w497
                  tunnel: w495 -> [w516]
                  frame #0 {
                    n261 = xnode "Read/Write Control"("FPGA VI Reference In"=w516, "Конфигурация"=TRUE) -> ("FPGA VI Reference Out"=w517:refnum<k20>)  [unwired: 1 in, 1 out]
                    n262 = Wait (ms)(milliseconds to wait=u32 10) -> ()  [unwired: 1 out]
                  }
                }
                n263 = flat-sequence {
                  tunnel: w497 -> [w514]
                  tunnel: [w512] -> w494
                  frame #0 {
                    n264 = xnode "Read/Write Control"("FPGA VI Reference In"=w514, "Конфигурация"=FALSE) -> ("FPGA VI Reference Out"=w512:refnum<k20>)  [unwired: 1 in, 1 out]
                    n265 = Wait (ms)(milliseconds to wait=u32 10) -> ()  [unwired: 1 out]
                  }
                }
                n266 = xnode "Read/Write Control"("FPGA VI Reference In"=w485, "error in"=w484) -> ("READ"=→"?":bool[])  [unwired: 2 out]
              }
              frame #3 {
                # "MUX"
                n267 = xnode "Read/Write Control"("FPGA VI Reference In"=w527, "Enum"=T8."MUX") -> ("FPGA VI Reference Out"=w521:refnum<k20>)  [unwired: 1 in, 1 out]
                n268 = xnode "Read/Write Control"("FPGA VI Reference In"=w520, "Read(T)/Write(F)"=TRUE) -> ("FPGA VI Reference Out"=w534:refnum<k20>, "error out"=w533:errorcluster)  [unwired: 1 in]
                n269 = xnode "Read/Write Control"("FPGA VI Reference In"=w521, "Read(T)/Write(F)"=FALSE) -> ("FPGA VI Reference Out"=w523:refnum<k20>)  [unwired: 1 in, 1 out]
                n270 = flat-sequence {
                  tunnel: w534 -> [w555]
                  tunnel: w533 -> [w554]
                  tunnel: [w553] -> w532
                  tunnel: [w552] -> w531
                  frame #0 {
                    n271 = xnode "Read/Write Control"("FPGA VI Reference In"=w555, "error in"=w554, "Конфигурация"=TRUE) -> ("FPGA VI Reference Out"=w553:refnum<k20>, "error out"=w552:errorcluster)
                    n272 = Wait (ms)(milliseconds to wait=u32 10) -> ()  [unwired: 1 out]
                  }
                }
                n273 = xnode "Read/Write Control"("FPGA VI Reference In"=w523, "Write Data"=bool[] [FALSE, TRUE, FALSE, TRUE, FALSE, FALSE, FALSE, FALSE, FALSE]) -> ("FPGA VI Reference Out"=w524:refnum<k20>)  [unwired: 1 in, 1 out]
                n274 = flat-sequence {
                  tunnel: w532 -> [w549]
                  tunnel: w531 -> [w548]
                  tunnel: [w546] -> w530
                  tunnel: [w545] -> w529
                  frame #0 {
                    n275 = xnode "Read/Write Control"("FPGA VI Reference In"=w549, "error in"=w548, "Конфигурация"=FALSE) -> ("FPGA VI Reference Out"=w546:refnum<k20>, "error out"=w545:errorcluster)
                    n276 = Wait (ms)(milliseconds to wait=u32 10) -> ()  [unwired: 1 out]
                  }
                }
                n277 = flat-sequence {
                  tunnel: [w542] -> w525
                  tunnel: w524 -> [w541]
                  frame #0 {
                    n278 = xnode "Read/Write Control"("FPGA VI Reference In"=w541, "Конфигурация"=TRUE) -> ("FPGA VI Reference Out"=w542:refnum<k20>)  [unwired: 1 in, 1 out]
                    n279 = Wait (ms)(milliseconds to wait=u32 10) -> ()  [unwired: 1 out]
                  }
                }
                n280 = flat-sequence {
                  tunnel: w525 -> [w539]
                  tunnel: [w537] -> w520
                  frame #0 {
                    n281 = xnode "Read/Write Control"("FPGA VI Reference In"=w539, "Конфигурация"=FALSE) -> ("FPGA VI Reference Out"=w537:refnum<k20>)  [unwired: 1 in, 1 out]
                    n282 = Wait (ms)(milliseconds to wait=u32 10) -> ()  [unwired: 1 out]
                  }
                }
                n283 = xnode "Read/Write Control"("FPGA VI Reference In"=w530, "error in"=w529) -> ("READ"=→"?":bool[])  [unwired: 2 out]
              }
            }
          }
        }
      }
      frame #2 {
        n284 = case shown="True" "?" {
          tunnel: w556 -> [w565 w575]
          tunnel: w563 -> [_ w574]
          tunnel: w562 -> [_ w573]
          tunnel: w561 -> [w567 w572]
          tunnel: [w567 w571] -> w560
          tunnel: [w566 w570] -> w559
          tunnel: w558 -> [w566 w569]
          frame False {
            n285 = xnode "Read/Write Control"("FPGA VI Reference In"=w565, "Кадр в память"=FALSE) -> ()  [unwired: 1 in, 2 out]
            n286 = Wait (ms)(milliseconds to wait=u32 5) -> ()  [unwired: 1 out]
          }
          frame True {
            n287 = stacked-sequence {
              seq-local: [_ _ w615 _] -> [_ _ _ w681]
              seq-local: [w579 _ _ _] -> [_ w587 _ _]
              tunnel: w575 -> [w577 w590 w612 w678]
              tunnel: w574 -> [_ _ w626 _]
              tunnel: w573 -> [_ _ w625 _]
              tunnel: w572 -> [_ _ _ w688]
              tunnel: [_ _ _ w685] -> w571
              tunnel: [_ _ _ w680] -> w570
              tunnel: w569 -> [_ _ w614 _]
              frame #0 {
                n288 = xnode "Read/Write Control"("FPGA VI Reference In"=w577, "Кадр в память"=FALSE) -> ()  [unwired: 1 in, 2 out]
                n289 = local write "Картинка"(FALSE ("Картинка")) -> ()
                n290 = xnode "Invoke Method"("FPGA VI Reference In"=w577, "Number of Elements"=u32 0, "Timeout (ms)"=0) -> ("FPGA VI Reference Out"=w582:refnum<k20>, "error out"=w581:errorcluster, "Elements Remaining"=w580:u32)  [unwired: 1 in, 1 out]
                n291 = xnode "Invoke Method"("FPGA VI Reference In"=w582, "error in"=w581, "Number of Elements"=w580) -> ("Data"=w579:u8[])  [unwired: 1 in, 3 out]
              }
              frame #1 {
                n292 = flat-sequence {
                  tunnel: w590 -> [w593]
                  tunnel: [w592] -> w588
                  tunnel: w587 -> [_]
                  tunnel: [w591] -> w586
                  tunnel: [w601] -> w589
                  tunnel: w588 -> [w602]
                  tunnel: w586 -> [w599]
                  tunnel: [w599] -> w585
                  tunnel: w589 -> [w604]
                  tunnel: w585 -> [w603]
                  frame #0 {
                    # "I"
                    n293 = while {
                      tunnel: w593 -> [w598]
                      tunnel: [w597] -> w592
                      tunnel: [w596] -> w591
                      stop <- w594 stop-if-true
                      n294 = xnode "Read/Write Control"("FPGA VI Reference In"=w598) -> ("FPGA VI Reference Out"=w597:refnum<k20>, "I"=w596:i32)  [unwired: 1 in, 1 out]
                      n295 = Equal?(x=w596, y=2022) -> (x = y?=w594:bool)
                    }
                  }
                  frame #1 {
                    n296 = xnode "Read/Write Control"("FPGA VI Reference In"=w602, "Кадр в память"=TRUE) -> ("FPGA VI Reference Out"=w601:refnum<k20>)  [unwired: 1 in, 1 out]
                  }
                  frame #2 {
                    # "I"
                    n297 = while {
                      tunnel: w604 -> [w609]
                      tunnel: [w605] -> _
                      tunnel: w603 -> [_]
                      stop <- w608 stop-if-true
                      n298 = xnode "Read/Write Control"("FPGA VI Reference In"=w609) -> ("FPGA VI Reference Out"=w605:refnum<k20>, "I"=w607:i32)  [unwired: 1 in, 1 out]
                      n299 = Equal?(x=w607, y=2020) -> (x = y?=w608:bool)
                    }
                  }
                }
              }
              frame #2 {
                # "L"
                # "H"
                # "2146304"
                n300 = for {
                  N: "?" -> [_]
                  tunnel: [w652] -> w627 mode=indexing
                  shift-right: [w649] -> _
                  shift-left: w626 -> [w651]
                  shift-right: [w648] -> _
                  shift-left: w625 -> [w650]
                  tunnel: w612 -> [w647]
                  n301 = stacked-sequence {
                    tunnel: [_ _ _ _ w667] -> w652
                    tunnel: w651 -> [w654 _ _ _ _]
                    tunnel: w650 -> [w655 _ _ _ _]
                    tunnel: [w657 _ _ _ _] -> w649
                    tunnel: [w656 _ _ _ _] -> w648
                    tunnel: w647 -> [w653 w659 w661 w663 w668]
                    frame #0 {
                      n302 = xnode "Read/Write Control"("FPGA VI Reference In"=w653, "Нач_адр"=w654, "Кон_адр"=w655) -> ()  [unwired: 1 in, 2 out]
                      n303 = local read "16384"() -> (w658:u32)
                      n304 = Add(x=w654, y=w658) -> (x+y=w657:u32)
                      n305 = Add(x=w658, y=w655) -> (x+y=w656:u32)
                    }
                    frame #1 {
                      n306 = xnode "Read/Write Control"("FPGA VI Reference In"=w659, "Кадр на ПК 16384"=TRUE ("HOST")) -> ()  [unwired: 1 in, 2 out]
                    }
                    frame #2 {
                      n307 = xnode "Read/Write Control"("FPGA VI Reference In"=w661, "Кадр на ПК 16384"=FALSE ("HOST")) -> ()  [unwired: 1 in, 2 out]
                    }
                    frame #3 {
                      n308 = while {
                        tunnel: w663 -> [w665]
                        stop <- w666 stop-if-true
                        # "Записан FIFO?"
                        n309 = xnode "Read/Write Control"("FPGA VI Reference In"=w665) -> ("Записали FIFO"=w666:bool)  [unwired: 1 in, 2 out]
                        n310 = Wait (ms)(milliseconds to wait=u32 1) -> ()  [unwired: 1 out]
                      }
                    }
                    frame #4 {
                      n311 = xnode "Invoke Method"("FPGA VI Reference In"=w668, "Number of Elements"=u32 0, "Timeout (ms)"=0) -> ("FPGA VI Reference Out"=w672:refnum<k20>, "Elements Remaining"=w673:u32)  [unwired: 1 in, 2 out]
                      n312 = xnode "Invoke Method"("FPGA VI Reference In"=w672, "Number of Elements"=w673, "Timeout (ms)"=0) -> ("Data"=w667:u8[])  [unwired: 1 in, 3 out]
                    }
                  }
                }
                n313 = xnode "Read/Write Control"("FPGA VI Reference In"=w612, "Кадр в память"=FALSE) -> ("FPGA VI Reference Out"=w611:refnum<k20>)  [unwired: 1 in, 1 out]
                n314 = Reshape Array(w627, 4292608 ("dimension size")) -> (w617:u8[])
                n315 = Reverse 1D Array(array=w617) -> (reversed array=w616:u8[])
                n316 = Decimate 1D Array(w616) -> (w619:u8[], w618:u8[])
                n317 = case shown="False" "?" {
                  tunnel: w619 -> [w633 w636]
                  tunnel: w618 -> [w634 w635]
                  tunnel: [w634 w636] -> w624
                  tunnel: [w633 w635] -> w623
                  tunnel: w611 -> [_ _]
                  frame False {
                  }
                  frame True {
                  }
                }
                n318 = for {
                  N: 2146304 -> [_]
                  tunnel: [w643] -> w610 mode=indexing
                  tunnel: w624 -> [w640]
                  tunnel: w623 -> [w639]
                  i -> [w646]
                  n319 = Index Array(array=w640, index=w646) -> (element=w638:u8)
                  n320 = Index Array(array=w639, index=w646) -> (element=w637:u8)
                  n321 = To Unsigned Word Integer(number=w638) -> (unsigned 16bit integer=w642:u16)
                  n322 = To Unsigned Word Integer(number=w637) -> (unsigned 16bit integer=w641:u16)
                  n323 = Multiply(x=w642, y=u16 256) -> (x*y=w644:u16)
                  n324 = Add(x=w644, y=w641) -> (x+y=w643:u16)
                }
                n325 = for {
                  tunnel: w614 -> [w632] mode=indexing
                  tunnel: w610 -> [w630] mode=indexing
                  tunnel: [w631] -> w615 mode=indexing
                  n326 = To Unsigned Quad Integer(1:w630) -> (0:w629:u64)
                  n327 = Add(x=w632, y=w629) -> (x+y=w631:u64)
                }
              }
              frame #3 {
                n328 = Increment(x=w688) -> (x+1=w687:u8)
                n329 = for {
                  tunnel: w681 -> [w696] mode=indexing
                  tunnel: "?" -> [w695]
                  tunnel: [w693] -> w676 mode=indexing
                  n330 = Divide(x=w696, y=w695) -> (x/y=w694:dbl)
                  n331 = To Unsigned Word Integer(number=w694) -> (unsigned 16bit integer=w693:u16)
                }
                n332 = Equal?(x=w687, y="?") -> (x = y?=w683:bool)
                n333 = xnode "Read/Write Control"("FPGA VI Reference In"=w678, "Кадр в память"=FALSE) -> ("FPGA VI Reference Out"=w677:refnum<k20>)  [unwired: 1 in, 1 out]
                n334 = Select(t=u8 0, s=w683, f=w687) -> (s? t:f=w685:u8)
                "?" <- w685
                n335 = case shown="True" w683 {
                  tunnel: w676 -> [_ w701]
                  tunnel: w677 -> [_ _]
                  frame False {
                  }
                  frame True {
                    w710 = T9 6 items=["Grayscale (U8)", "Grayscale (I16)", "Grayscale (SGL)", "Complex (CSG)", "RGB (U32)", "HSL (U32)", "RGB (U64)"] ("Image Type")
                    n336 = Multiply(x=w701, y="?") -> (x*y=w702:u16[])
                    n337 = for {
                      N: "?" -> [_]
                      shift-right: [w719] -> _
                      shift-left: w702 -> [w720]
                      tunnel: [w721] -> w706 mode=indexing
                      n338 = Delete From Array(array=w720, length="?", index=0) -> (deleted portion=w721:u16[], array with subset deleted=w719:u16[])
                    }
                    n339 = local write "Получить кадр"(FALSE ("Получить средний кадр")) -> ()
                    n340 = call "IMAQ Create"("Image Name"="FPPZ1024", "Image Type"=w710) -> ("New Image"=w709:T7)  [unwired: 3 in, 1 out]
                    n341 = for {
                      N: 2146304 -> [_]
                      tunnel: [w713] -> w703 mode=indexing
                      i -> [w713]
                    }
                    n342 = for {
                      N: 2048 -> [_]
                      tunnel: [w716] -> w699 mode=indexing
                      tunnel: w706 -> [w715] mode=indexing
                      n343 = for {
                        N: 1032 -> [_]
                        tunnel: [w718] -> w716 mode=indexing
                        tunnel: w715 -> [w717] mode=indexing
                        n344 = Bundle(w717, w717, w717, w717) -> (w718:cluster{u16, u16, u16, u16})  [unwired: 1 in]
                      }
                    }
                    "?" <- w699
                    n345 = call "IMAQ ArrayToColorImage"("Image"=w709, "Image Pixels (U64)"=w699) -> ("Image Out"=w697:T7)  [unwired: 3 in, 1 out]
                    "?" <- w697
                    n346 = flat-sequence {
                      tunnel: w697 -> [_]
                      frame #0 {
                        "?" <- TRUE ("Картинка")
                      }
                    }
                    n347 = Bundle(w703, w702) -> (→"?":cluster{i32[], u16[]})  [unwired: 1 in]
                  }
                }
                n348 = Select(t=u64[] array[2146304 elements], s=w683, f=w681) -> (s? t:f=w680:u64[])
                n349 = case shown="True" "?" {
                  tunnel: w676 -> [_ w690]
                  tunnel: "?" -> [_ w689]
                  frame False {
                  }
                  frame True {
                    n350 = case shown="\"1 кадр\", Default" w689 {
                      tunnel: w690 -> [w691 w692]
                      frame "1 кадр", Default {
                        "?" <- w691
                      }
                      frame "2 кадр" {
                        "?" <- w692
                      }
                    }
                  }
                }
              }
            }
          }
        }
      }
      frame #3 {
        n351 = xnode "Read/Write Control"("FPGA VI Reference In"=w726, "Остановка основного цикла"="?") -> ("FPGA VI Reference Out"=w725:refnum<k20>)  [unwired: 1 in, 1 out]
        n352 = case shown="True" "?" {
          frame False {
          }
          frame True {
            n353 = local write "Линейки"(FALSE ("Линейки")) -> ()
          }
        }
      }
    }
  }
  n354 = while {
    tunnel: w18 -> [w735]
    tunnel: w17 -> [w730]
    tunnel: w16 -> [w729]
    tunnel: [w734] -> w15
    tunnel: [w733] -> w14
    tunnel: [w732] -> w13
    stop <- w728 stop-if-true
    n355 = Wait (ms)(milliseconds to wait=u32 2) -> ()  [unwired: 1 out]
    n356 = stacked-sequence {
      seq-local: [w736 _] -> [_ w738]
      tunnel: w735 -> [_ w772]
      tunnel: [_ w771] -> w734
      tunnel: [_ w770] -> w733
      tunnel: [_ w769] -> w732
      tunnel: w730 -> [_ w756]
      tunnel: w729 -> [_ w743]
      tunnel: [_ w738] -> w728
      frame #0 {
        n357 = local read "Стоп"() -> (w736:bool)
      }
      frame #1 {
        w742 = T10 0 items=["Current", "Voltage"] ("measurement type")
        # "STAB +15"
        # "STAB -15"
        # "STAB +15"
        # "12"
        # "STEP"
        # "REL"
        # "5"
        # "5"
        # "5"
        # "ADC_D"
        # "ADC_A"
        n358 = Not(x=w738) -> (.not. x?=w740:bool)
        n359 = And(x=w740, y="?") -> (x .and. y?=w741:bool)
        n360 = call <instrlib>:"niDCPower Configure Current Limit.vi"("current limit"="?", "channel name"="0", "instrument handle"=w743) -> ("instrument handle out"=w807:refnum<k15>)  [unwired: 7 in, 1 out]
        n361 = call <instrlib>:"niDCPower Configure Current Limit.vi"("current limit"="?", "channel name"="1", "instrument handle"=w743) -> ("instrument handle out"=w808:refnum<k15>)  [unwired: 7 in, 1 out]
        n362 = call <instrlib>:"niDCPower Configure Current Limit.vi"("current limit"="?", "channel name"="1", "instrument handle"=w756) -> ("instrument handle out"=w809:refnum<k15>)  [unwired: 7 in, 1 out]
        n363 = call <instrlib>:"niDCPower Configure Current Limit.vi"("current limit"="?", "channel name"="2", "instrument handle"=w756) -> ("instrument handle out"=w810:refnum<k15>)  [unwired: 7 in, 1 out]
        n364 = call <instrlib>:"niDCPower Configure Current Limit.vi"("current limit"="?", "channel name"="0", "instrument handle"=w772) -> ("instrument handle out"=w811:refnum<k15>)  [unwired: 7 in, 1 out]
        n365 = call <instrlib>:"niDCPower Configure Current Limit.vi"("current limit"="?", "channel name"="1", "instrument handle"=w772) -> ("instrument handle out"=w812:refnum<k15>)  [unwired: 7 in, 1 out]
        n366 = call <instrlib>:"niDCPower Configure Current Limit.vi"("current limit"="?", "channel name"="0", "instrument handle"=w756) -> ("instrument handle out"=w762:refnum<k15>)  [unwired: 7 in, 1 out]
        n367 = call <instrlib>:"niDCPower Configure Current Limit.vi"("current limit"="?", "channel name"="2", "instrument handle"=w743) -> ("instrument handle out"=w750:refnum<k15>)  [unwired: 7 in, 1 out]
        n368 = call <instrlib>:"niDCPower Configure Voltage Level.vi"("voltage level"="?", "channel name"="1", "instrument handle"=w809) -> ("error out"=w790:errorcluster, "instrument handle out"=w787:refnum<k15>)  [unwired: 7 in]
        n369 = call <instrlib>:"niDCPower Configure Voltage Level.vi"("voltage level"="?", "channel name"="2", "instrument handle"=w810) -> ("error out"=w789:errorcluster, "instrument handle out"=w788:refnum<k15>)  [unwired: 7 in]
        n370 = call <instrlib>:"niDCPower Configure Voltage Level.vi"("voltage level"="?", "channel name"="0", "instrument handle"=w811) -> ("error out"=w799:errorcluster, "instrument handle out"=w802:refnum<k15>)  [unwired: 7 in]
        n371 = call <instrlib>:"niDCPower Configure Voltage Level.vi"("voltage level"="?", "channel name"="1", "instrument handle"=w812) -> ("error out"=w800:errorcluster, "instrument handle out"=w801:refnum<k15>)  [unwired: 7 in]
        n372 = call <instrlib>:"niDCPower Configure Voltage Level.vi"("voltage level"="?", "channel name"="0", "instrument handle"=w807) -> ("error out"=w777:errorcluster, "instrument handle out"=w780:refnum<k15>)  [unwired: 7 in]
        n373 = call <instrlib>:"niDCPower Configure Voltage Level.vi"("voltage level"="?", "channel name"="1", "instrument handle"=w808) -> ("error out"=w778:errorcluster, "instrument handle out"=w779:refnum<k15>)  [unwired: 7 in]
        n374 = call <instrlib>:"niDCPower Configure Voltage Level.vi"("voltage level"="?", "channel name"="0", "instrument handle"=w762) -> ("error out"=w766:errorcluster, "instrument handle out"=w767:refnum<k15>)  [unwired: 7 in]
        n375 = call <instrlib>:"niDCPower Configure Voltage Level.vi"("voltage level"="?", "channel name"="2", "instrument handle"=w750) -> ("error out"=w753:errorcluster, "instrument handle out"=w752:refnum<k15>)  [unwired: 7 in]
        n376 = call <instrlib>:"niDCPower Configure Output Enabled.vi"("error in (no error)"=w790, "output enabled"=w741, "channel name"="1", "instrument handle"=w787) -> ("error out"=w836:errorcluster, "instrument handle out"=w829:refnum<k15>)  [unwired: 6 in]
        n377 = call <instrlib>:"niDCPower Configure Output Enabled.vi"("error in (no error)"=w789, "output enabled"=w741, "channel name"="2", "instrument handle"=w788) -> ("error out"=w831:errorcluster, "instrument handle out"=w830:refnum<k15>)  [unwired: 6 in]
        n378 = call <instrlib>:"niDCPower Configure Output Enabled.vi"("error in (no error)"=w799, "output enabled"=w741, "channel name"="0", "instrument handle"=w802) -> ("error out"=w833:errorcluster, "instrument handle out"=w832:refnum<k15>)  [unwired: 6 in]
        n379 = call <instrlib>:"niDCPower Configure Output Enabled.vi"("error in (no error)"=w800, "output enabled"=w741, "channel name"="1", "instrument handle"=w801) -> ("error out"=w834:errorcluster, "instrument handle out"=w835:refnum<k15>)  [unwired: 6 in]
        n380 = call <instrlib>:"niDCPower Configure Output Enabled.vi"("error in (no error)"=w777, "output enabled"=w741, "channel name"="0", "instrument handle"=w780) -> ("error out"=w820:errorcluster, "instrument handle out"=w819:refnum<k15>)  [unwired: 6 in]
        n381 = call <instrlib>:"niDCPower Configure Output Enabled.vi"("error in (no error)"=w778, "output enabled"=w741, "channel name"="1", "instrument handle"=w779) -> ("error out"=w821:errorcluster, "instrument handle out"=w822:refnum<k15>)  [unwired: 6 in]
        n382 = call <instrlib>:"niDCPower Configure Output Enabled.vi"("error in (no error)"=w766, "output enabled"=w741, "channel name"="0", "instrument handle"=w767) -> ("error out"=w758:errorcluster, "instrument handle out"=w759:refnum<k15>)  [unwired: 6 in]
        n383 = call <instrlib>:"niDCPower Configure Output Enabled.vi"("error in (no error)"=w753, "output enabled"="?", "channel name"="2", "instrument handle"=w752) -> ("error out"=w748:errorcluster, "instrument handle out"=w747:refnum<k15>)  [unwired: 6 in]
        n384 = call <instrlib>:"niDCPower Measure.vi"("error in (no error)"=w820, "measurement type"=w742, "channel name"="0", "instrument handle"=w819) -> ("measurement"=→"?":dbl, "instrument handle out"=w771:refnum<k15>)  [unwired: 5 in, 1 out]
        n385 = call <instrlib>:"niDCPower Measure.vi"("error in (no error)"=w821, "measurement type"=w742, "channel name"="1", "instrument handle"=w822) -> ("measurement"=→"?":dbl)  [unwired: 5 in, 2 out]
        n386 = call <instrlib>:"niDCPower Measure.vi"("error in (no error)"=w836, "measurement type"=w742, "channel name"="1", "instrument handle"=w829) -> ("measurement"=→"?":dbl, "instrument handle out"=w770:refnum<k15>)  [unwired: 5 in, 1 out]
        n387 = call <instrlib>:"niDCPower Measure.vi"("error in (no error)"=w831, "measurement type"=w742, "channel name"="2", "instrument handle"=w830) -> ("measurement"=→"?":dbl)  [unwired: 5 in, 2 out]
        n388 = call <instrlib>:"niDCPower Measure.vi"("error in (no error)"=w758, "measurement type"=w742, "channel name"="0", "instrument handle"=w759) -> ("measurement"=→"?":dbl)  [unwired: 5 in, 2 out]
        n389 = call <instrlib>:"niDCPower Measure.vi"("error in (no error)"=w748, "measurement type"=w742, "channel name"="2", "instrument handle"=w747) -> ("measurement"=→"?":dbl)  [unwired: 5 in, 2 out]
        n390 = call <instrlib>:"niDCPower Measure.vi"("error in (no error)"=w833, "measurement type"=w742, "channel name"="0", "instrument handle"=w832) -> ("measurement"=→"?":dbl, "instrument handle out"=w769:refnum<k15>)  [unwired: 5 in, 1 out]
        n391 = call <instrlib>:"niDCPower Measure.vi"("error in (no error)"=w834, "measurement type"=w742, "channel name"="1", "instrument handle"=w835) -> ("measurement"=→"?":dbl)  [unwired: 5 in, 2 out]
      }
    }
  }
  n392 = while {
    tunnel: w3 -> [w847]
    shift-right: [w845] -> _
    shift-left: _ -> [w846]
    stop <- w849 stop-if-true
    n393 = stacked-sequence {
      tunnel: [_ _ _ w938] -> w849
      tunnel: w847 -> [_ w889 _ _]
      tunnel: w846 -> [w852 _ _ _]
      tunnel: [w851 _ _ _] -> w845
      frame #0 {
        # "Проверка токов на тиристоры"
        n394 = local read "Питание"() -> (w851:bool)
        n395 = Greater?(x=w851, y=w852) -> (0:w850:bool)
        n396 = flat-sequence {
          tunnel: w850 -> [w853]
          frame #0 {
            n397 = case shown="True" w853 {
              frame False {
              }
              frame True {
                n398 = stacked-sequence {
                  frame #0 {
                    n399 = Wait (ms)(milliseconds to wait=u32 500) -> ()  [unwired: 1 out]
                  }
                  frame #1 {
                    n400 = flat-sequence {
                      frame #0 {
                        n401 = local write "Прошить АЦП"(TRUE ("Прошить АЦП")) -> ()
                        n402 = Wait (ms)(milliseconds to wait=u32 25) -> ()  [unwired: 1 out]
                      }
                      frame #1 {
                        n403 = local write "Прошить АЦП"(FALSE ("Прошить АЦП")) -> ()
                        n404 = Wait (ms)(milliseconds to wait=u32 25) -> ()  [unwired: 1 out]
                      }
                    }
                  }
                }
              }
            }
          }
          frame #1 {
            n405 = local read "STAB_+15_cur"() -> (w867:dbl)
            n406 = local read "STAB_-15_cur"() -> (w864:dbl)
            n407 = local read "STEP_cur"() -> (w861:dbl)
            n408 = Greater?(x=w861, y="?") -> (0:w859:bool)
            "?" <- w859
            n409 = Greater?(x=w867, y="?") -> (0:w865:bool)
            "?" <- w865
            n410 = Greater?(x=w864, y="?") -> (0:w862:bool)
            "?" <- w862
            n411 = case shown="True" w865 {
              frame False {
              }
              frame True {
                n412 = local read "STAB_+15"() -> (w873:i32)
                n413 = Increment(x=w873) -> (x+1=→"?":i32)
              }
            }
            n414 = case shown="True" w862 {
              frame False {
              }
              frame True {
                n415 = local read "STAB_-15"() -> (w870:i32)
                n416 = Increment(x=w870) -> (x+1=→"?":i32)
              }
            }
            n417 = case shown="True" w859 {
              frame False {
              }
              frame True {
                n418 = local read "STEP"() -> (w869:i32)
                n419 = Increment(x=w869) -> (x+1=→"?":i32)
              }
            }
          }
        }
      }
      frame #1 {
        w876 = i16 0 ("width (-)")
        w879 = i16 7 ("width (-)")
        w905 = i16 7 ("width (-)")
        w906 = i16 3 ("width (-)")
        w907 = i16 0 ("width (-)")
        w908 = i16 3 ("width (-)")
        w878 = "\t"
        # "Логирование данных"
        n420 = local read "ADC_A_cur"() -> (w925:dbl)
        n421 = local read "ADC_D_cur"() -> (w924:dbl)
        n422 = local read "TEMP_cur"() -> (w923:dbl)
        n423 = local read "LED_cur"() -> (w922:dbl)
        n424 = local read "REL_cur"() -> (w921:dbl)
        n425 = local read "STAB_+15_cur"() -> (w920:dbl)
        n426 = local read "STAB_+15"() -> (w919:i32)
        n427 = local read "18_cur"() -> (w914:dbl)
        n428 = local read "28_cur"() -> (w913:dbl)
        n429 = local read "STAB_-15_cur"() -> (w918:dbl)
        n430 = local read "STAB_-15"() -> (w917:i32)
        n431 = local read "STEP_cur"() -> (w916:dbl)
        n432 = local read "STEP"() -> (w915:i32)
        n433 = Number To Fractional String(number=w925, width (-)=w908, precision (6)=w908) -> (F-format string=w904:string)  [unwired: 1 in]
        n434 = Number To Fractional String(number=w924, width (-)=w908, precision (6)=w908) -> (F-format string=w903:string)  [unwired: 1 in]
        n435 = Number To Fractional String(number=w923, width (-)=w908, precision (6)=w908) -> (F-format string=w902:string)  [unwired: 1 in]
        n436 = Number To Fractional String(number=w922, width (-)=w908, precision (6)=w908) -> (F-format string=w901:string)  [unwired: 1 in]
        n437 = Number To Fractional String(number=w921, width (-)=w908, precision (6)=w908) -> (F-format string=w900:string)  [unwired: 1 in]
        n438 = Number To Fractional String(number=w920, width (-)=w908, precision (6)=w908) -> (F-format string=w899:string)  [unwired: 1 in]
        n439 = Number To Fractional String(number=w919, width (-)=w907, precision (6)=w907) -> (F-format string=w898:string)  [unwired: 1 in]
        n440 = Number To Fractional String(number=w918, width (-)=w906, precision (6)=w906) -> (F-format string=w897:string)  [unwired: 1 in]
        n441 = Number To Fractional String(number=w917, width (-)=w907, precision (6)=w907) -> (F-format string=w896:string)  [unwired: 1 in]
        n442 = Number To Fractional String(number=w916, width (-)=w906, precision (6)=w906) -> (F-format string=w895:string)  [unwired: 1 in]
        n443 = Number To Fractional String(number=w915, width (-)=w907, precision (6)=w907) -> (F-format string=w894:string)  [unwired: 1 in]
        n444 = Number To Fractional String(number=w914, width (-)=w879, precision (6)=w879) -> (F-format string=w893:string)  [unwired: 1 in]
        n445 = Number To Fractional String(number=w913, width (-)=w879, precision (6)=w879) -> (F-format string=w892:string)  [unwired: 1 in]
        n446 = Get Date/Time In Seconds() -> (seconds since 1Jan1904=w928:timestamp)
        n447 = Format Date/Time String(time format string (%c)="%d %H:%M:%S:%3u", seconds (now)=w928) -> (date/time string=w926:string)  [unwired: 1 in]
        n448 = local read "30_cur"() -> (w909:dbl)
        n449 = Number To Fractional String(number=w909, width (-)=w905, precision (6)=w905) -> (F-format string=w891:string)  [unwired: 1 in]
        n450 = Select(t="О", s="?", f="") -> (s? t:f=w890:string)
        n451 = local read "Промеры"() -> (w877:i32)
        n452 = local read "STAB_+15"() -> (w887:bool)
        n453 = local read "STAB_-15"() -> (w888:bool)
        n454 = local read "SIM_SEL"() -> (w885:bool)
        n455 = local read "STEP"() -> (w886:bool)
        n456 = Number To Fractional String(number=w877, width (-)=w876, precision (6)=w876) -> (F-format string=w875:string)  [unwired: 1 in]
        n457 = Compound Arithmetic op=OR(w888, w887, w886, w885) -> (w884:bool)
        n458 = Select(t="!!!", s=w884, f="") -> (s? t:f=w880:string)
        n459 = Concatenate Strings(w926, w878, w904, w878, w903, w878, w902, w878, w901, w878, w900, w878, w899, w878, w898, w878, w897, w878, w896, w878, w895, w878, w894, w878, w893, w878, w892, w878, w891, w878, w890, w878, w880, w878, w878, w875, "\r\n") -> (w927:string)
        n460 = Format Into String(initial string=w889, w927) -> ()  [unwired: 2 in, 2 out]
      }
      frame #2 {
        n461 = local read "STAB_+15"() -> (w931:bool)
        n462 = local read "STAB_-15"() -> (w932:bool)
        n463 = local read "STEP"() -> (w930:bool)
        n464 = Compound Arithmetic op=OR(w932, w931, w930, "?") -> (w933:bool)
        n465 = case shown="True" w933 {
          frame False {
          }
          frame True {
            n466 = flat-sequence {
              frame #0 {
                n467 = local write "Питание"(FALSE ("Питание")) -> ()
              }
              frame #1 {
                n468 = Wait (ms)(milliseconds to wait="?") -> ()  [unwired: 1 out]
              }
              frame #2 {
                n469 = local write "Питание"(TRUE ("Питание")) -> ()
              }
              frame #3 {
                n470 = Wait (ms)(milliseconds to wait=u32 200) -> ()  [unwired: 1 out]
              }
            }
          }
        }
      }
      frame #3 {
        n471 = local read "Стоп"() -> (w938:bool)
      }
    }
    n472 = Wait (ms)(milliseconds to wait=u32 2) -> ()  [unwired: 1 out]
  }
  n473 = while {
    tunnel: w6 -> [w947]
    tunnel: w5 -> [w946]
    shift-right: [w944] -> _
    shift-left: _ -> [w945]
    tunnel: [w943] -> w4
    shift-right: [w939] -> _
    shift-left: 0 -> [w940]
    stop <- w942 stop-if-true
    n474 = stacked-sequence {
      tunnel: w947 -> [w953 _]
      tunnel: w946 -> [w952 w1061]
      tunnel: w945 -> [w951 _]
      tunnel: ["?" _] -> w944
      tunnel: [_ w1061] -> w943
      tunnel: [_ w1060] -> w942
      tunnel: w940 -> [w949 _]
      tunnel: [w948 _] -> w939
      frame #0 {
        # "Работа с реле и вывод промеренных токов"
        n475 = Greater?(x="?", y=w951) -> (0:w954:bool)
        n476 = case shown="True" w954 {
          tunnel: w953 -> [_ w960]
          tunnel: w952 -> [_ w959]
          tunnel: w949 -> [w955 w958]
          tunnel: [w955 w957] -> w948
          frame False {
            n477 = Wait (ms)(milliseconds to wait=u32 10) -> ()  [unwired: 1 out]
          }
          frame True {
            n478 = stacked-sequence {
              tunnel: w960 -> [w972 w1007 w1036]
              tunnel: w959 -> [w971 w1006 w1035]
              tunnel: w958 -> [w966 _ _]
              tunnel: [w964 _ _] -> w957
              frame #0 {
                # "Промер цепи 18"
                n479 = flat-sequence {
                  tunnel: w972 -> [w978]
                  tunnel: [w977] -> w970
                  tunnel: w966 -> [w973]
                  tunnel: [w973] -> w965
                  tunnel: w970 -> [w985]
                  tunnel: [w984] -> w969
                  tunnel: w965 -> [w980]
                  tunnel: [w979] -> w961
                  tunnel: w971 -> [w990]
                  tunnel: w969 -> [w988]
                  tunnel: [w988] -> w968
                  tunnel: [w986] -> w962
                  tunnel: w961 -> [w986]
                  tunnel: w968 -> [w996]
                  tunnel: [w994] -> w967
                  tunnel: [w991] -> w963
                  tunnel: w962 -> [w991]
                  tunnel: w967 -> [w1001]
                  tunnel: [w997] -> w964
                  tunnel: w963 -> [w997]
                  frame #0 {
                    # "Подключить \nк амперметру"
                    n480 = xnode "Read/Write Control"("FPGA VI Reference In"=w978, "RELAY_18_IN1"=FALSE, "RELAY_18_IN2"=TRUE) -> ("FPGA VI Reference Out"=w977:refnum<k20>)  [unwired: 1 in, 1 out]
                    n481 = Wait (ms)(milliseconds to wait=u32 50) -> ()  [unwired: 1 out]
                  }
                  frame #1 {
                    # "Отключить\nцепь"
                    n482 = Wait (ms)(milliseconds to wait=u32 50) -> ()  [unwired: 1 out]
                    n483 = xnode "Read/Write Control"("FPGA VI Reference In"=w985, "RELAY_18_IN1"=TRUE, "RELAY_18_IN2"=TRUE) -> ("FPGA VI Reference Out"=w984:refnum<k20>)  [unwired: 1 in, 1 out]
                    n484 = Increment(x=w980) -> (x+1=w979:i32)
                  }
                  frame #2 {
                    n485 = call <instrlib>:"niDMM Read.vi"("instrument handle"=w990) -> ("Measurement"=→"?":dbl)  [unwired: 8 in, 2 out]
                    n486 = Wait (ms)(milliseconds to wait=u32 50) -> ()  [unwired: 1 out]
                  }
                  frame #3 {
                    # "Подключить\nцепь"
                    n487 = xnode "Read/Write Control"("FPGA VI Reference In"=w996, "RELAY_18_IN1"=FALSE, "RELAY_18_IN2"=TRUE) -> ("FPGA VI Reference Out"=w994:refnum<k20>)  [unwired: 1 in, 1 out]
                    n488 = Wait (ms)(milliseconds to wait=u32 50) -> ()  [unwired: 1 out]
                  }
                  frame #4 {
                    # "Отключить \nамперметр"
                    n489 = xnode "Read/Write Control"("FPGA VI Reference In"=w1001, "RELAY_18_IN1"=FALSE, "RELAY_18_IN2"=FALSE) -> ()  [unwired: 1 in, 2 out]
                    n490 = Wait (ms)(milliseconds to wait=u32 50) -> ()  [unwired: 1 out]
                  }
                }
              }
              frame #1 {
                # "Промер цепи 28"
                n491 = flat-sequence {
                  tunnel: w1007 -> [w1012]
                  tunnel: [w1011] -> w1005
                  tunnel: w1005 -> [w1017]
                  tunnel: [w1016] -> w1004
                  tunnel: w1006 -> [w1021]
                  tunnel: w1004 -> [w1019]
                  tunnel: [w1019] -> w1003
                  tunnel: w1003 -> [w1026]
                  tunnel: [w1024] -> w1002
                  tunnel: w1002 -> [w1030]
                  frame #0 {
                    # "Подключить \nк амперметру"
                    n492 = xnode "Read/Write Control"("FPGA VI Reference In"=w1012, "RELAY_28_IN1"=FALSE, "RELAY_28_IN2"=TRUE) -> ("FPGA VI Reference Out"=w1011:refnum<k20>)  [unwired: 1 in, 1 out]
                    n493 = Wait (ms)(milliseconds to wait=u32 50) -> ()  [unwired: 1 out]
                  }
                  frame #1 {
                    # "Отключить\nцепь"
                    n494 = Wait (ms)(milliseconds to wait=u32 50) -> ()  [unwired: 1 out]
                    n495 = xnode "Read/Write Control"("FPGA VI Reference In"=w1017, "RELAY_28_IN1"=TRUE, "RELAY_28_IN2"=TRUE) -> ("FPGA VI Reference Out"=w1016:refnum<k20>)  [unwired: 1 in, 1 out]
                  }
                  frame #2 {
                    n496 = call <instrlib>:"niDMM Read.vi"("instrument handle"=w1021) -> ("Measurement"=→"?":dbl)  [unwired: 8 in, 2 out]
                    n497 = Wait (ms)(milliseconds to wait=u32 50) -> ()  [unwired: 1 out]
                  }
                  frame #3 {
                    # "Подключить\nцепь"
                    n498 = xnode "Read/Write Control"("FPGA VI Reference In"=w1026, "RELAY_28_IN1"=FALSE, "RELAY_28_IN2"=TRUE) -> ("FPGA VI Reference Out"=w1024:refnum<k20>)  [unwired: 1 in, 1 out]
                    n499 = Wait (ms)(milliseconds to wait=u32 50) -> ()  [unwired: 1 out]
                  }
                  frame #4 {
                    # "Отключить \nамперметр"
                    n500 = xnode "Read/Write Control"("FPGA VI Reference In"=w1030, "RELAY_28_IN1"=FALSE, "RELAY_28_IN2"=FALSE) -> ()  [unwired: 1 in, 2 out]
                    n501 = Wait (ms)(milliseconds to wait=u32 50) -> ()  [unwired: 1 out]
                  }
                }
              }
              frame #2 {
                # "Промер цепи 30"
                n502 = flat-sequence {
                  tunnel: w1036 -> [w1041]
                  tunnel: [w1040] -> w1034
                  tunnel: w1034 -> [w1046]
                  tunnel: [w1045] -> w1033
                  tunnel: w1035 -> [w1050]
                  tunnel: w1033 -> [w1048]
                  tunnel: [w1048] -> w1032
                  tunnel: w1032 -> [w1055]
                  tunnel: [w1053] -> w1031
                  tunnel: w1031 -> [w1059]
                  frame #0 {
                    # "Подключить \nк амперметру"
                    n503 = xnode "Read/Write Control"("FPGA VI Reference In"=w1041, "RELAY_30_IN1"=FALSE, "RELAY_30_IN2"=TRUE) -> ("FPGA VI Reference Out"=w1040:refnum<k20>)  [unwired: 1 in, 1 out]
                    n504 = Wait (ms)(milliseconds to wait=u32 50) -> ()  [unwired: 1 out]
                  }
                  frame #1 {
                    # "Отключить\nцепь"
                    n505 = xnode "Read/Write Control"("FPGA VI Reference In"=w1046, "RELAY_30_IN1"=TRUE, "RELAY_30_IN2"=TRUE) -> ("FPGA VI Reference Out"=w1045:refnum<k20>)  [unwired: 1 in, 1 out]
                    n506 = Wait (ms)(milliseconds to wait=u32 50) -> ()  [unwired: 1 out]
                  }
                  frame #2 {
                    n507 = call <instrlib>:"niDMM Read.vi"("instrument handle"=w1050) -> ("Measurement"=→"?":dbl)  [unwired: 8 in, 2 out]
                    n508 = Wait (ms)(milliseconds to wait=u32 50) -> ()  [unwired: 1 out]
                  }
                  frame #3 {
                    # "Подключить\nцепь"
                    n509 = xnode "Read/Write Control"("FPGA VI Reference In"=w1055, "RELAY_30_IN1"=FALSE, "RELAY_30_IN2"=TRUE) -> ("FPGA VI Reference Out"=w1053:refnum<k20>)  [unwired: 1 in, 1 out]
                    n510 = Wait (ms)(milliseconds to wait=u32 50) -> ()  [unwired: 1 out]
                  }
                  frame #4 {
                    # "Отключить \nамперметр"
                    n511 = xnode "Read/Write Control"("FPGA VI Reference In"=w1059, "RELAY_30_IN1"=FALSE, "RELAY_30_IN2"=FALSE) -> ()  [unwired: 1 in, 2 out]
                    n512 = Wait (ms)(milliseconds to wait=u32 50) -> ()  [unwired: 1 out]
                  }
                }
              }
            }
          }
        }
        "?" <- w948
      }
      frame #1 {
        n513 = local read "Стоп"() -> (w1060:bool)
      }
    }
    n514 = Wait (ms)(milliseconds to wait=u32 20) -> ()  [unwired: 1 out]
  }
  n515 = call <instrlib>:"niDCPower Close.vi"("instrument handle"=w15) -> ()  [unwired: 10 in, 1 out]
  n516 = call <instrlib>:"niDCPower Close.vi"("instrument handle"=w14) -> ()  [unwired: 10 in, 1 out]
  n517 = call <instrlib>:"niDCPower Close.vi"("instrument handle"=w13) -> ()  [unwired: 10 in, 1 out]
  n518 = xnode "Invoke Method"("FPGA VI Reference In"=w12) -> ()  [unwired: 1 in, 2 out]
  n519 = call <instrlib>:"niDMM Close.vi"("instrument handle"=w4) -> ()  [unwired: 10 in, 1 out]
